vi "UI Main.vi"() -> ()   [LabVIEW 2025]
uses:
  support/User Event - Stop/User Event - Stop.lvlib
  controls/UI Data.ctl
  support/Message Queue/Message Queue.lvlib
  Globals/Global - All UI Loop Stop.vi
  Globals/Global - Configuration Options.vi
  controls/Control State.ctl
  controls/Raw Values.ctl
  controls/Control Configuration.ctl
  controls/All Control Configuration Values.ctl
  Globals/Global - UI Stream and Variable Connections.vi
  Globals/ALL MCS Registers.vi
  5TR Lab/5TR Lab/Global Variables/cRIO channels Input.vi
  <vilib>/numeric/Random Number (Range) U64.vi
  C:/40T/controls/ProfiBusData.ctl
  controls/Profi address.ctl
  controls/Tempratures.ctl
  controls/Power Meters.ctl
  controls/Unit Temp.ctl
  controls/Main UI.ctl
panel:
  in  "Controller Address 2":string
  in  "Hc0 3":i32(listbox)
  in  "Seek Forward Button":bool
  in  "数据列表 2":enum32{"40TR", "Chiller"}(tab)
  in  "Tab Control 2":T1(tab)
  in  "Cluster":T2
  in  "Cluster 2":T3
  in  "ID_HEATER_Stage_3":bool
  in  "ID_HEATER_Stage_2":bool
  in  "OD_HEATER_Stage_1":bool
  in  "ID_HEATER_Stage_3":bool
  in  "ID_HEATER_Stage_2":bool
  in  "Cluster 3":T4
  in  "AUX Chiller Pump_ 2":bool
  in  "AUX Chiller Pump_1":bool
  in  "Hc0 2":i32(listbox)
  in  "Hc1 2":i32(listbox)
  in  "Forget Password":bool
  in  "Add paramter":bool
  in  "数据列表":enum32{"40TR", "Chiller"}(tab)
  in  "Hc0":i32(listbox)
  in  "Hc1":i32(listbox)
  out "WIKA Temprature Transmitters 2":T5
  out "WIKA Temprature Transmitters":T6
  out "Temp":T7
  out "AO1":dbl
  in  "Cluster 4":cluster{"Play Button":bool, "Pause Button":bool}
  in  "Stop Button 2":bool
  in  "Stop Button":bool
  in  "Main System":T8(tab)
  in  "Power":bool
  in  "New User":bool
  in  "Login":bool
  in  "Account":enum16{"AMTECH", "Admin", "Operator"}(ring)=enum."Admin"
  in  "Password":string
  in  "Name":string
  in  "Tab Control":T9(tab)
  in  "Main Configuration":T10={"Unit Model "="", "Reported by"="", "Test Standard"="", "Tested by"="", "Job Number"="NA", "Test Facility"="40TR-Lab", "Power Supply"="", "Other:    PS"="", "Unit Family"="Package", "Requester"="ENG", "Client "="", "Project"="", "Serial Number"="", "Brand"="", "Manufacturer"="", "Test Type"="Package"}
  out "Performed Tests":string[](array[string])
  in  "Load input parameters":bool
  in  "Start Runing":bool
  out "Refrigrant":sgl=98.71708 format="%#.2f"
  out "Ambient_Temp L 2":sgl=98.71708 format="%#.2f"
  out "Ambient_Temp R 2":sgl=98.71708 format="%#.2f"
  out "Coil":sgl=98.71708 format="%#.2f"
  out "Refrigrant Press Tempratures":T11
  out "Ambient R Grid TEMPERATURE  Grid":T12
  out "Ambient L Grid TEMPERATURE Grid":T13
  out "ON-COIL TEMPERATURE  Grid":T12
  out "OFF-COIL TEMPERATURE Grid":T13
  out "Ambient_Temp L":sgl=98.71708 format="%#.2f"
  out "Ambient_Temp R":sgl=98.71708 format="%#.2f"
  out "Ambient":sgl=98.71708 format="%#.2f"
  in  "Save config":bool
  in  "Pressure":T15(array[cluster])
  in  "Power Meters":cluster{"Profi":T14, "Name":T16}[](array[cluster])
  in  "Tempratures":cluster{"Name":T17, "Profi":T14, "Unit":T18}[][](array[cluster])
  out "Main UI":T19
  in  "chiller lab":T20(tab)
  in  "Exit":bool
  out "Control Input Values Crio1":T21(graph)
  out "Control Output Values":T22(graph)
  out "CPU Usage crio2 (%) 2":dbl(graph)
  out "Low Speed Loop Period (ms)":u32
  out "Control Loop Period (ms)":u32
  out "Largest Contiguous Memory (bytes)":dbl(graph)
  out "CPU Usage crio1 (%)":dbl(graph)
  in  "Stop Control":bool
  in  "Run Control":bool
  in  "Control Configurations":T23[](array[typedef])
  in  "Update Control Configuration":bool
  out "Channel 0 Setpoint":dbl
  out "Channel 1 Setpoint":dbl
  out "Channel 2 Setpoint":dbl
  out "Channel 3 Setpoint":dbl
  in  "Temperature Thresholds":dbl[](array[numeric])
  out "Control INputs Crio2":T24(graph)
  in  "Switch to Safe State":bool
  out "System Status":string
  out "Current Control Mode":u16(ring) items=["Safe State", "Control (PID)"]
  out "Connected?":bool
  in  "Connect to Controller":bool
  in  "Controller Address":string
  # "Sensor O/P Values"
  # "Sensor I/P Readings"
  # "LabVIEW Real-Time Control on CompactRIO (RIO Scan Interface)"
  # "Connection Settings"
  # "R"
  # "L"
  # "ON"
  # "OFF"
  # "Element 0 - Chan 0\nElement 1 - Chan 1\nElement 2 - Chan 2\nElement 3 - Chan 3"
  # "Setpoint changes are sent to the target automatically."
  # "Note: In order to set manual outputs in the control loop, you can force IO values through the NI Distributed System Manager, available by right-clicking the CompactRIO target in the project and choosing Utilities > View in System Manager."
  # "Control Configuration changes are sent to the target when you click \"Update Control Configurations\"."
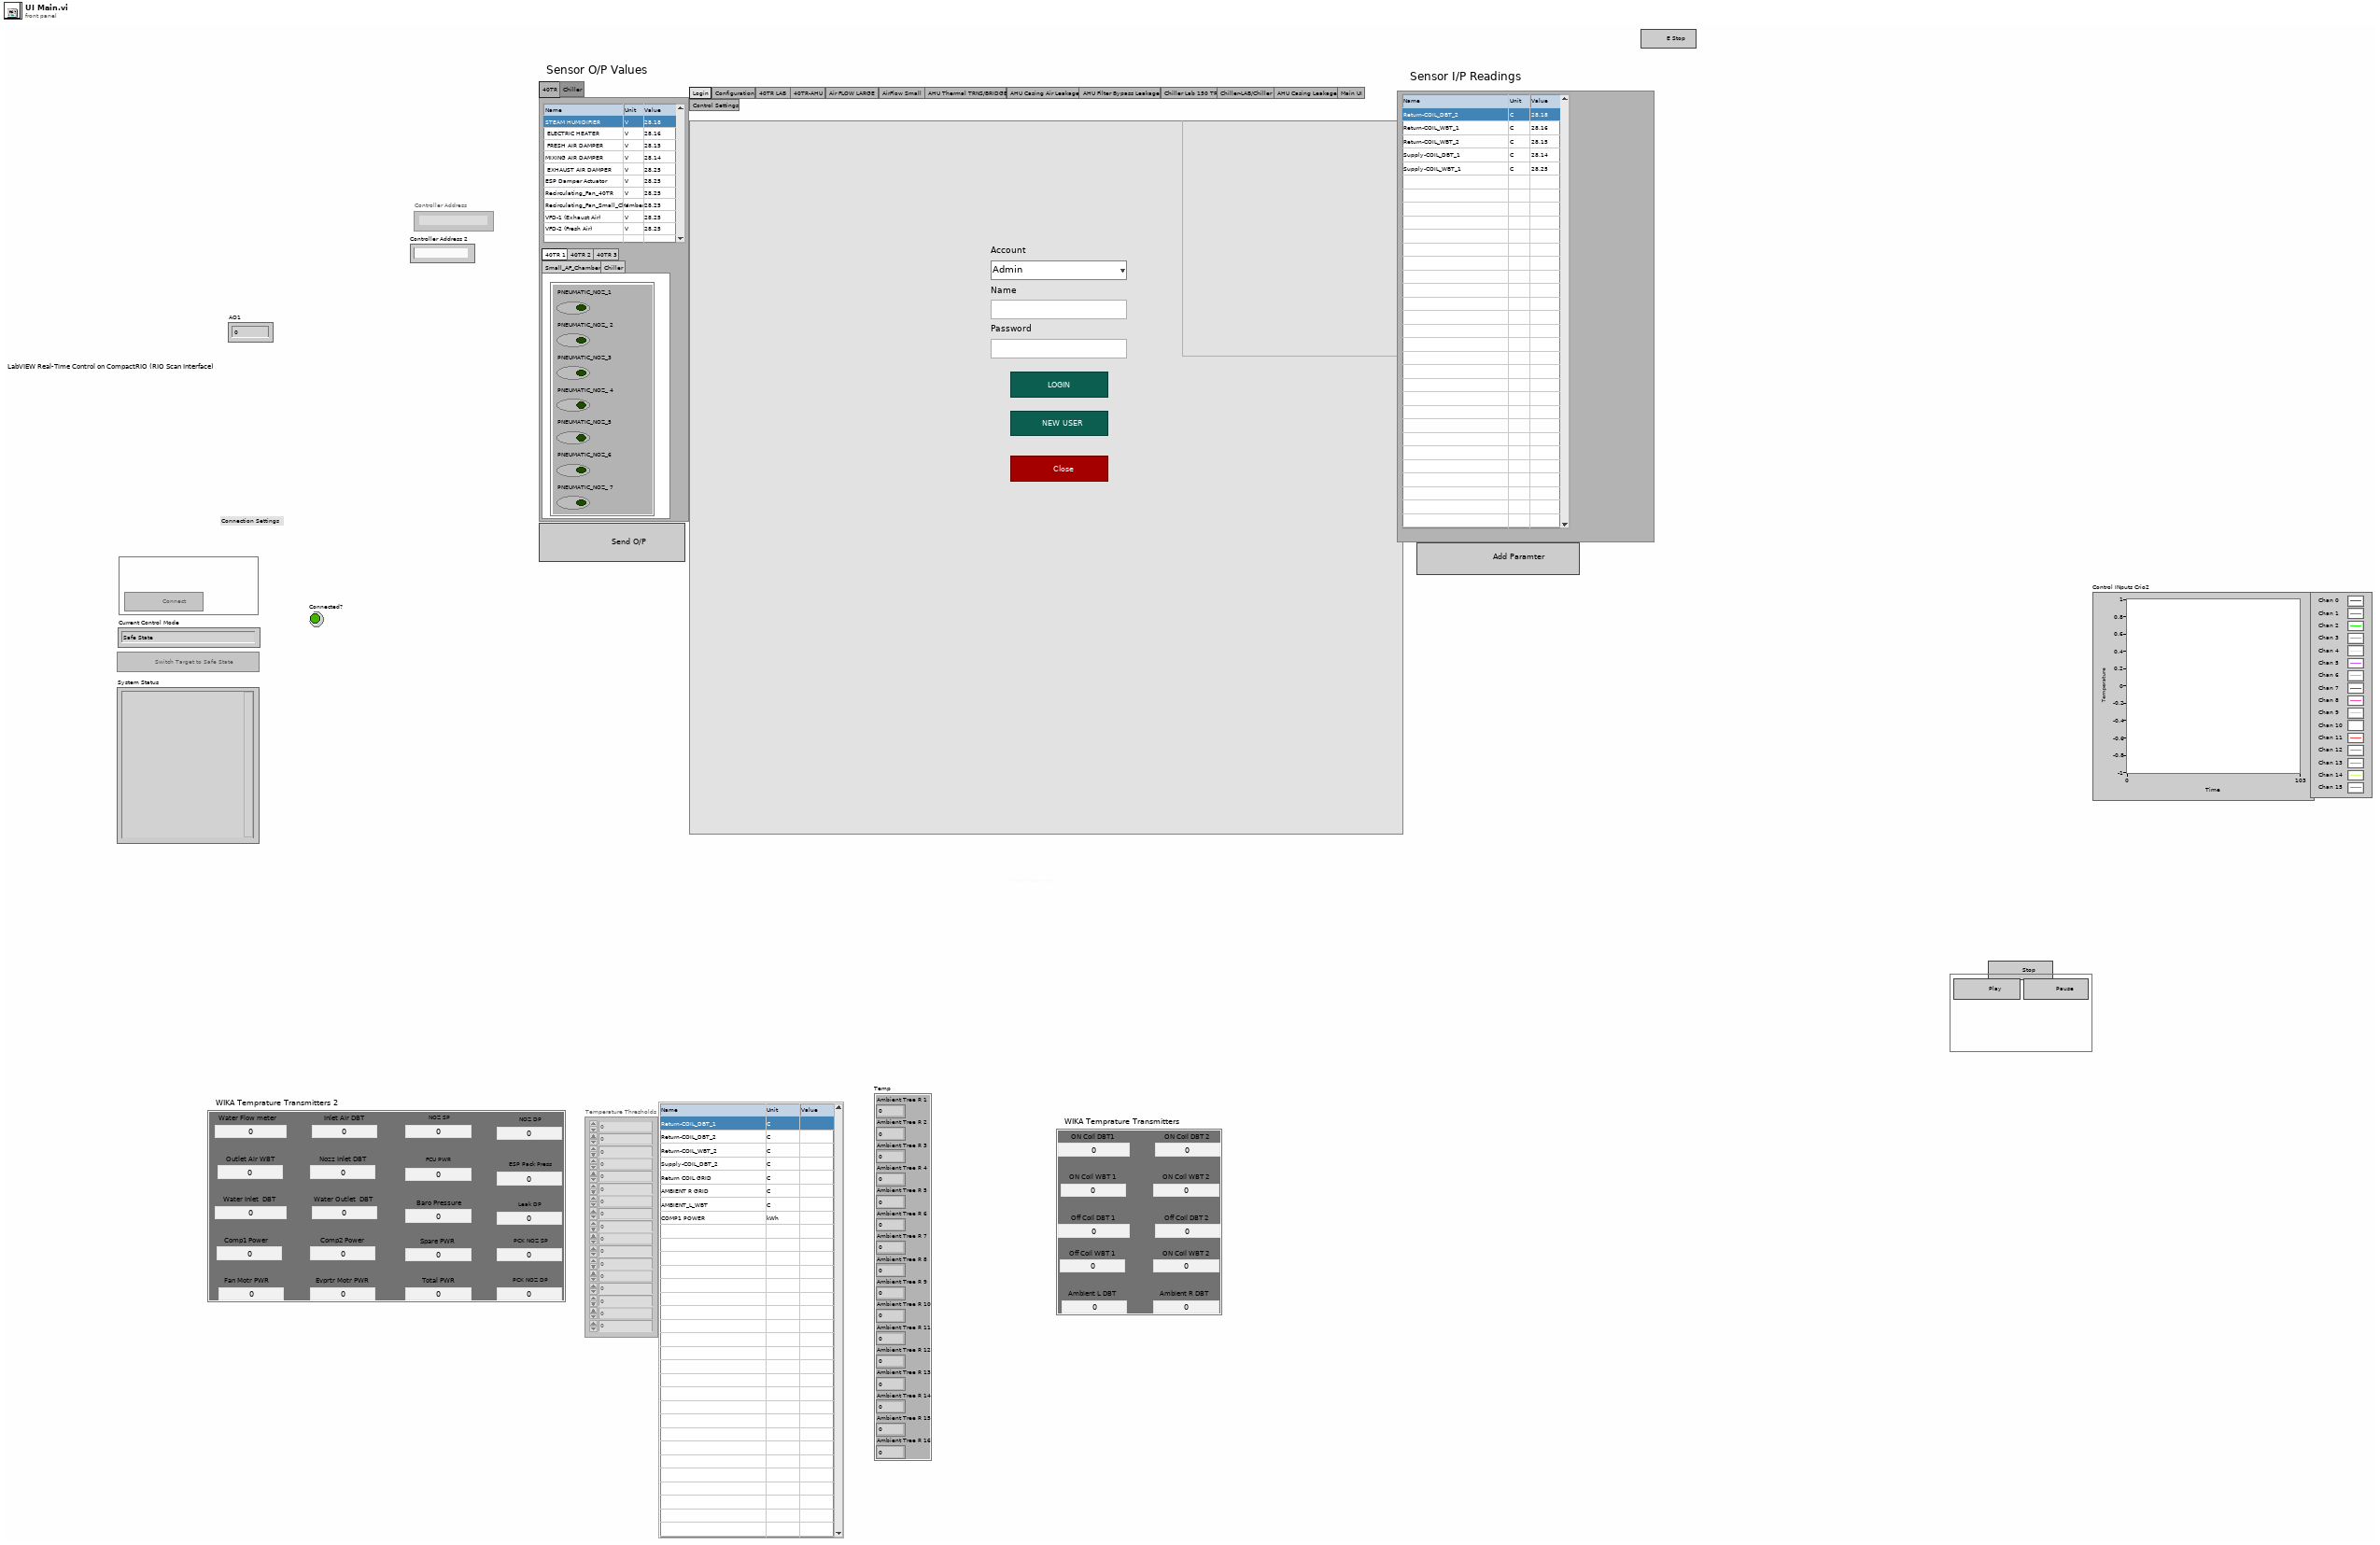
[diagram p1: front panel]
types:
  T1 = enum32{"40TR 1", "40TR 2", "40TR 3", "Small_AF_Chamber", "Chiller"}
  T2 = cluster{"PNEUMATIC_NOZ_1":bool, "PNEUMATIC_NOZ_ 2":bool, "PNEUMATIC_NOZ_3":bool, "PNEUMATIC_NOZ_ 4":bool, "PNEUMATIC_NOZ_5":bool, "PNEUMATIC_NOZ_6":bool, "PNEUMATIC_NOZ_ 7":bool}
  T3 = cluster{"Recirculating_Fan_40TR":bool, "Recirculating_Fan_40TR 2":bool, "STEAM HUMIDIFIER":bool, "VFD-2 (Exahust Air)":bool, "VFD-2 (Fresh Air) ":bool, "VFD_Fan_Leak_setup":bool, "ID_HEATER_Stage_1":bool}
  T4 = cluster{"PNEUMATIC_NOZ_1":bool, "PNEUMATIC_NOZ_ 2":bool, "PNEUMATIC_NOZ_3":bool, "PNEUMATIC_NOZ_ 4":bool, "PNEUMATIC_NOZ_5":bool}
  T5 = cluster{"Water Flow meter":dbl, "Inlet Air DBT ":dbl, "Outlet Air WBT ":dbl, "Nozz Inlet DBT":dbl, "Water Outlet  DBT ":dbl, "Water Inlet  DBT ":dbl, "Comp1 Power":dbl, "Comp2 Power":dbl, "Fan Motr PWR":dbl, "Evprtr Motr PWR":dbl, "Total PWR ":dbl, "Spare PWR":dbl, "Baro Pressure":dbl, "FCU PWR":dbl, "NOZ SP":dbl, "NOZ DP":dbl, "ESP Pack Press":dbl, "Leak DP":dbl, "PCK NOZ SP":dbl, "PCK NOZ DP":dbl}
  T6 = cluster{"ON Coil DBT1  ":dbl, "ON Coil DBT 2":dbl, "ON Coil WBT 1":dbl, "ON Coil WBT 2":dbl, "Off Coil DBT 2":dbl, "Off Coil DBT 1":dbl, "Off Coil WBT 1":dbl, "ON Coil WBT 2":dbl, "Ambient L DBT":dbl, "Ambient R DBT":dbl}
  T7 = cluster{"Ambient Tree R 1":dbl, "Ambient Tree R 2":dbl, "Ambient Tree R 3":dbl, "Ambient Tree R 4":dbl, "Ambient Tree R 5":dbl, "Ambient Tree R 6":dbl, "Ambient Tree R 7":dbl, "Ambient Tree R 8":dbl, "Ambient Tree R 9":dbl, "Ambient Tree R 10":dbl, "Ambient Tree R 11":dbl, "Ambient Tree R 12":dbl, "Ambient Tree R 13":dbl, "Ambient Tree R 14":dbl, "Ambient Tree R 15":dbl, "Ambient Tree R 16":dbl}
  T8 = enum32{"Login", "Configuration", "40TR LAB ", "40TR-AHU", "Air FLOW LARGE", "AirFlow Small ", "AHU Thermal TRNS/BRIDGE", "AHU Casing Air Leakage", "AHU Filter Bypass Leakage ", "Chiller Lab 150 TR", "Chiller-LAB/Chiller", "AHU Casing Leakage", "Main UI", "Control Settings"}
  T9 = enum32{"Input Parameters", "All MCS DATA", "Assigned Sensors Profibus", "Ambient Trees", "Ternds"}
  T10 = cluster{"Unit Model ":string, "Reported by":string, "Test Standard":string, "Tested by":string, "Job Number":string, "Test Facility":string, "Power Supply":string, "Other:    PS":string, "Unit Family":string, "Requester":string, "Client ":string, "Project":string, "Serial Number":string, "Brand":string, "Manufacturer":string, "Test Type":string}
  T11 = cluster{"OFF Coil 1":dbl, "OFF Coil 2":dbl, "OFF Coil 3":dbl, "OFF Coil 4":dbl, "OFF Coil 5":dbl, "OFF Coil 6":dbl, "OFF Coil 7":dbl, "OFF Coil 8":dbl, "OFF Coil 9":dbl, "OFF Coil 10":dbl, "OFF Coil 11":dbl, "OFF Coil 12":dbl, "OFF Coil 13":dbl, "OFF Coil 14":dbl, "OFF Coil 15":dbl, "OFF Coil 16":dbl, "OFF Coil 17":dbl, "OFF Coil 18":dbl, "OFF Coil 19":dbl, "OFF Coil 20":dbl, "OFF Coil 21":dbl, "OFF Coil 22":dbl, "OFF Coil 23":dbl, "OFF Coil 24":dbl, "OFF Coil 25":dbl, "OFF Coil 26":dbl, "OFF Coil 27":dbl, "OFF Coil 28":dbl, "OFF Coil 29":dbl, "OFF Coil 30":dbl, "OFF Coil 31":dbl, "OFF Coil 32":dbl}
  T12 = cluster{"OFF Coil 1":dbl, "OFF Coil 2":dbl, "OFF Coil 3":dbl, "OFF Coil 4":dbl, "OFF Coil 5":dbl, "OFF Coil 6":dbl, "OFF Coil 7":dbl, "OFF Coil 8":dbl, "OFF Coil 9":dbl, "OFF Coil 10":dbl, "OFF Coil 11":dbl, "OFF Coil 12":dbl, "OFF Coil 13":dbl, "OFF Coil 14":dbl, "OFF Coil 15":dbl, "OFF Coil 16":dbl}
  T13 = cluster{"OFF Coil 1":dbl, "OFF Coil 2":dbl, "OFF Coil 3":dbl, "OFF Coil 4":dbl, "OFF Coil 5":dbl, "OFF Coil 6":dbl, "OFF Coil 7":dbl, "OFF Coil 8":dbl, "OFF Coil 9":dbl, "OFF Coil 10":dbl, "OFF Coil 11":dbl, "OFF Coil 12":dbl}
  T14 = typedef "Profi address.ctl" = string
  T15 = cluster{"Profi":T14, "Name":string, "Unit":string}[]
  T16 = typedef "Power Meters.ctl" = string
  T17 = typedef "Tempratures.ctl" = string
  T18 = typedef "Unit Temp.ctl" = string
  T19 = typedef "Main UI.ctl" = cluster{"Baro":dbl, "DBT On Coil":dbl, "WBT On Coil  ":dbl, "DBT Off  Coil ":dbl, "WBT Off Coil    ":dbl, "Noz Tem":dbl, "Noz  SP  49":dbl, "Noz  DP 50":dbl, "Nozzels":cluster{"Noz1":bool, "Noz 2":bool, "Noz 3":bool, "Noz 4":bool, "Noz 5":bool, "Noz 6":bool, "Noz 7":bool}, "ESP":dbl, "ESPDamper":dbl, "Humidifier":dbl, "Ambient Temp":cluster{"L_DBT":dbl, "R_DBT":dbl, "L_WBT":dbl, "R_WBT  ":dbl}, "Nozzels 2":cluster{"Ambient R":bool, "Ambient L":bool}, "Nozzels 3":cluster{"Return":bool}, "Cluster":cluster{"Supply":bool}, "40 TR":dbl, "E Air damper":dbl, "Mixed AD":dbl, "Fresh Air Dammper":dbl, "Nozzels 4":cluster{"VFD 1":dbl, "VFD 2":dbl}, "Nozzels 5":cluster{"OD-Heater1":bool, "OD-Heater 2":bool, "OD-Heater 3":bool}, "Consedate Weight":dbl, "Power Meter":cluster{"Comp1":dbl, "Comp2":dbl, "Cond Fan":dbl, "Ev-Motor":dbl, "Total":dbl, "Spare":dbl}}
  T20 = enum32{"UUT Water LOOP", "Cond -Coils Loop", "AUX Loop ", "Chiller Lab", "Data Monitoring", "System Monitoring"}
  T21 = cluster{"Control Input Values[0]":dbl, "Control Input Values[1]":dbl, "Control Input Values[2]":dbl, "Control Input Values[3]":dbl}
  T22 = cluster{"Control Output Values[0]":dbl, "Control Output Values[1]":dbl, "Control Output Values[2]":dbl, "Control Output Values[3]":dbl}
  T23 = typedef "Control Configuration.ctl" = cluster{"PID Gains":cluster{"proportional gain (Kc)":dbl, "integral gain (Kc*Ts/Ti)":dbl, "derivative gain (Kc*Td/Ts)":dbl}, "Output Range":cluster{"output high":dbl, "output low":dbl}}
  T24 = cluster{"Temperature Values[0]":dbl, "Temperature Values[1]":dbl, "Temperature Values[2]":dbl, "Temperature Values[3]":dbl, "Temperature Values[4]":dbl, "Temperature Values[5]":dbl, "Temperature Values[6]":dbl, "Temperature Values[7]":dbl, "Temperature Values[8]":dbl, "Temperature Values[9]":dbl, "Temperature Values[10]":dbl, "Temperature Values[11]":dbl, "Temperature Values[12]":dbl, "Temperature Values[13]":dbl, "Temperature Values[14]":dbl, "Temperature Values[15]":dbl}
  T25 = enum32{"UUT Water LOOP", "Cond -Coils Loop", "AUX Loop ", "Data Monitoring", "System Monitoring"}
  T26 = enum32{"Control Settings", "Chiller-LAB/Chiller", "40TR LAB ", "Page 2"}
  T27 = typedef "UI Data.ctl" = cluster{"Switch to Safe State Ref":refnum<vi>, "Run Control Ref":refnum<vi>, "Stop Control Ref":refnum<vi>, "Update Control Configurations Ref":refnum<vi>, "Ch 0 Setpoint Ref":refnum<vi>, "Ch 1 Setpoint Ref":refnum<vi>, "Ch 2 Setpoint Ref":refnum<vi>, "Ch 3 Setpoint Ref":refnum<vi>, "Control Configurations Ref":refnum<vi>, "Temperature Thresholds Ref":refnum<vi>}
  T28 = typedef "Message Queue.lvlib/All Message Queues.ctl" = cluster{"UI":refnum<queue>}
  T29 = cluster{"Room DP":dbl, "Barometric Pressure":dbl, "ID Nozzle DP":dbl, "OD Nozzle DP":dbl, "OD UUT Discharge Pressure":dbl, "OD UUT Suction Pressure":dbl, "OD UUT Liquid Pressure":dbl, "ID Humidifier Weight ":dbl, "ID UUT Condensate Weight":dbl, "ID Coil Condensate Weight":dbl, "OD Coil Water flow rate":dbl, "ID Flow Meter Channel":dbl}
  T30 = cluster{"ID UUT inlet DBT":dbl, "ID UUT inlet WBT":dbl, "ID UUT Outlet DBT":dbl, "OD UUT Outlet DBT":dbl, "ID UUT OUTLET WBT":dbl, "OD UUT INLET DBT":dbl, "OD UUT INLET WBT":dbl, "ID_EWT":dbl, "ID_LWT":dbl, "ID_Nozz_Temp":dbl}
  T31 = cluster{"ESP":dbl, "SP":dbl, "DP":dbl, "FCU WFR":dbl, "FCU Water PD":dbl, "RFM (lb/h)":dbl}
  T32 = cluster{"ON Coil 1":dbl, "ON Coil 2":dbl, "ON Coil 3":dbl, "ON Coil 4":dbl, "ON Coil 5":dbl, "ON Coil 6":dbl, "ON Coil 7":dbl, "ON Coil 8":dbl, "ON Coil 9":dbl, "ON Coil 10":dbl, "ON Coil 11":dbl, "ON Coil 12":dbl, "ON Coil 13":dbl, "ON Coil 14":dbl, "ON Coil 15":dbl, "ON Coil 16":dbl}
  T33 = cluster{"Ambient Tree L 1":dbl, "Ambient Tree L 2":dbl, "Ambient Tree L 3":dbl, "Ambient Tree L 4":dbl, "Ambient Tree L 5":dbl, "Ambient Tree L 6":dbl, "Ambient Tree L 7":dbl, "Ambient Tree L 8":dbl, "Ambient Tree L 9":dbl, "Ambient Tree L 10":dbl, "Ambient Tree L 11":dbl, "Ambient Tree L 12":dbl}
  T34 = typedef "Variable References.ctl" = cluster{"CPU Usage":refnum<k21>, "Contiguous Memory":refnum<k21>, "Control Mode":refnum<k21>, "Control Loop Period":refnum<k21>, "Low Speed Loop Period":refnum<k21>, "CPU Usage crio 2":refnum<k21>}
  T35 = typedef "IO References.ctl" = cluster{"Control Input Values":refnum<k21>[], "Control Output Values":refnum<k21>[], "Temperature Values":refnum<k21>[], "Threshold Exceeded":refnum<k21>, "Control Input Values 2":refnum<k21>[], "Control Output Values 2":refnum<k21>[], "Control Digital Values":refnum<k21>[], "Control Digital Values 2":refnum<k21>[]}
  T36 = typedef "Control State.ctl" = enum16{"Safe State", "Control (PID)"}
  T37 = cluster{"Control Input Values crio1 [0]":dbl, "Control Input Values crio1 [1]":dbl, "Control Input Values crio1 [2]":dbl, "Control Input Values crio1 [3]":dbl}
  T38 = cluster{"Input Values Crio2[0]":dbl, "Input Values Crio2[1]":dbl, "Input Values Crio2[2]":dbl, "Input Values Crio2[3]":dbl, "Input Values Crio2[4]":dbl, "Input Values Crio2[5]":dbl, "Input Values Crio2[6]":dbl, "Input Values Crio2[7]":dbl, "Input Values Crio2[8]":dbl, "Input Values Crio2[9]":dbl, "Input Values Crio2[10]":dbl, "Input Values Crio2[11]":dbl, "Input Values Crio2[12]":dbl, "Input Values Crio2[13]":dbl, "Input Values Crio2[14]":dbl, "Input Values Crio2[15]":dbl}
  T39 = typedef "ProfiBusData.ctl" = cluster{"[0]":dbl, "[1]":dbl, "[2]":dbl, "[3]":dbl, "[4]":dbl, "[5]":dbl, "[6]":dbl, "[7]":dbl, "[8]":dbl, "[9]":dbl, "[10]":dbl, "[11]":dbl, "[12]":dbl, "[13]":dbl, "[14]":dbl, "[15]":dbl, "[16]":dbl, "[17]":dbl, "[18]":dbl, "[19]":dbl, "[20]":dbl, "[21]":dbl, "[22]":dbl, "[23]":dbl, "[24]":dbl, "[25]":dbl, "[26]":dbl, "[27]":dbl, "[28]":dbl, "[29]":dbl, "[30]":dbl, "[31]":dbl, "[32]":dbl, "[33]":dbl, "[34]":dbl, "[35]":dbl, "[36]":dbl, "[37]":dbl, "[38]":dbl, "[39]":dbl, "[40]":dbl, "[41]":dbl, "[42]":dbl, "[43]":dbl, "[44]":dbl, "[45]":dbl, "[46]":dbl, "[47]":dbl, "[48]":dbl, "[49]":dbl, "[50]":dbl, "[51]":dbl, "[52]":dbl, "[53]":dbl, "[54]":dbl, "[55]":dbl, "[56]":dbl, "[57]":dbl, "[58]":dbl, "[59]":dbl, "[60]":dbl, "[61]":dbl, "[62]":dbl, "[63]":dbl, "[64]":dbl, "[65]":dbl, "[66]":dbl, "[67]":dbl, "[68]":dbl, "[69]":dbl, "[70]":dbl, "[71]":dbl, "[72]":dbl, "[73]":dbl, "[74]":dbl, "[75]":dbl, "[76]":dbl, "[77]":dbl, "[78]":dbl, "[79]":dbl, "[80]":dbl, "[81]":dbl, "[82]":dbl, "[83]":dbl, "[84]":dbl, "[85]":dbl, "[86]":dbl, "[87]":dbl, "[88]":dbl, "[89]":dbl, "[90]":dbl, "[91]":dbl, "[92]":dbl, "[93]":dbl, "[94]":dbl, "[95]":dbl, "[96]":dbl, "[97]":dbl, "[98]":dbl, "[99]":dbl, "[100]":dbl, "[101]":dbl, "[102]":dbl, "[103]":dbl, "[104]":dbl, "[105]":dbl, "[106]":dbl, "[107]":dbl, "[108]":dbl, "[109]":dbl, "[110]":dbl, "[111]":dbl, "[112]":dbl}
  T40 = cluster{"Message":string, "Message Data":variant}
  T41 = typedef "All Control Configuration Values.ctl" = cluster{"Control State":T36, "Setpoints":T42, "Control Configurations":T23[], "Temperature Thresholds":dbl[]}
  T42 = typedef "Raw Values.ctl" = cluster{"Channel 0":dbl, "Channel 1":dbl, "Channel 2":dbl, "Channel 3":dbl}
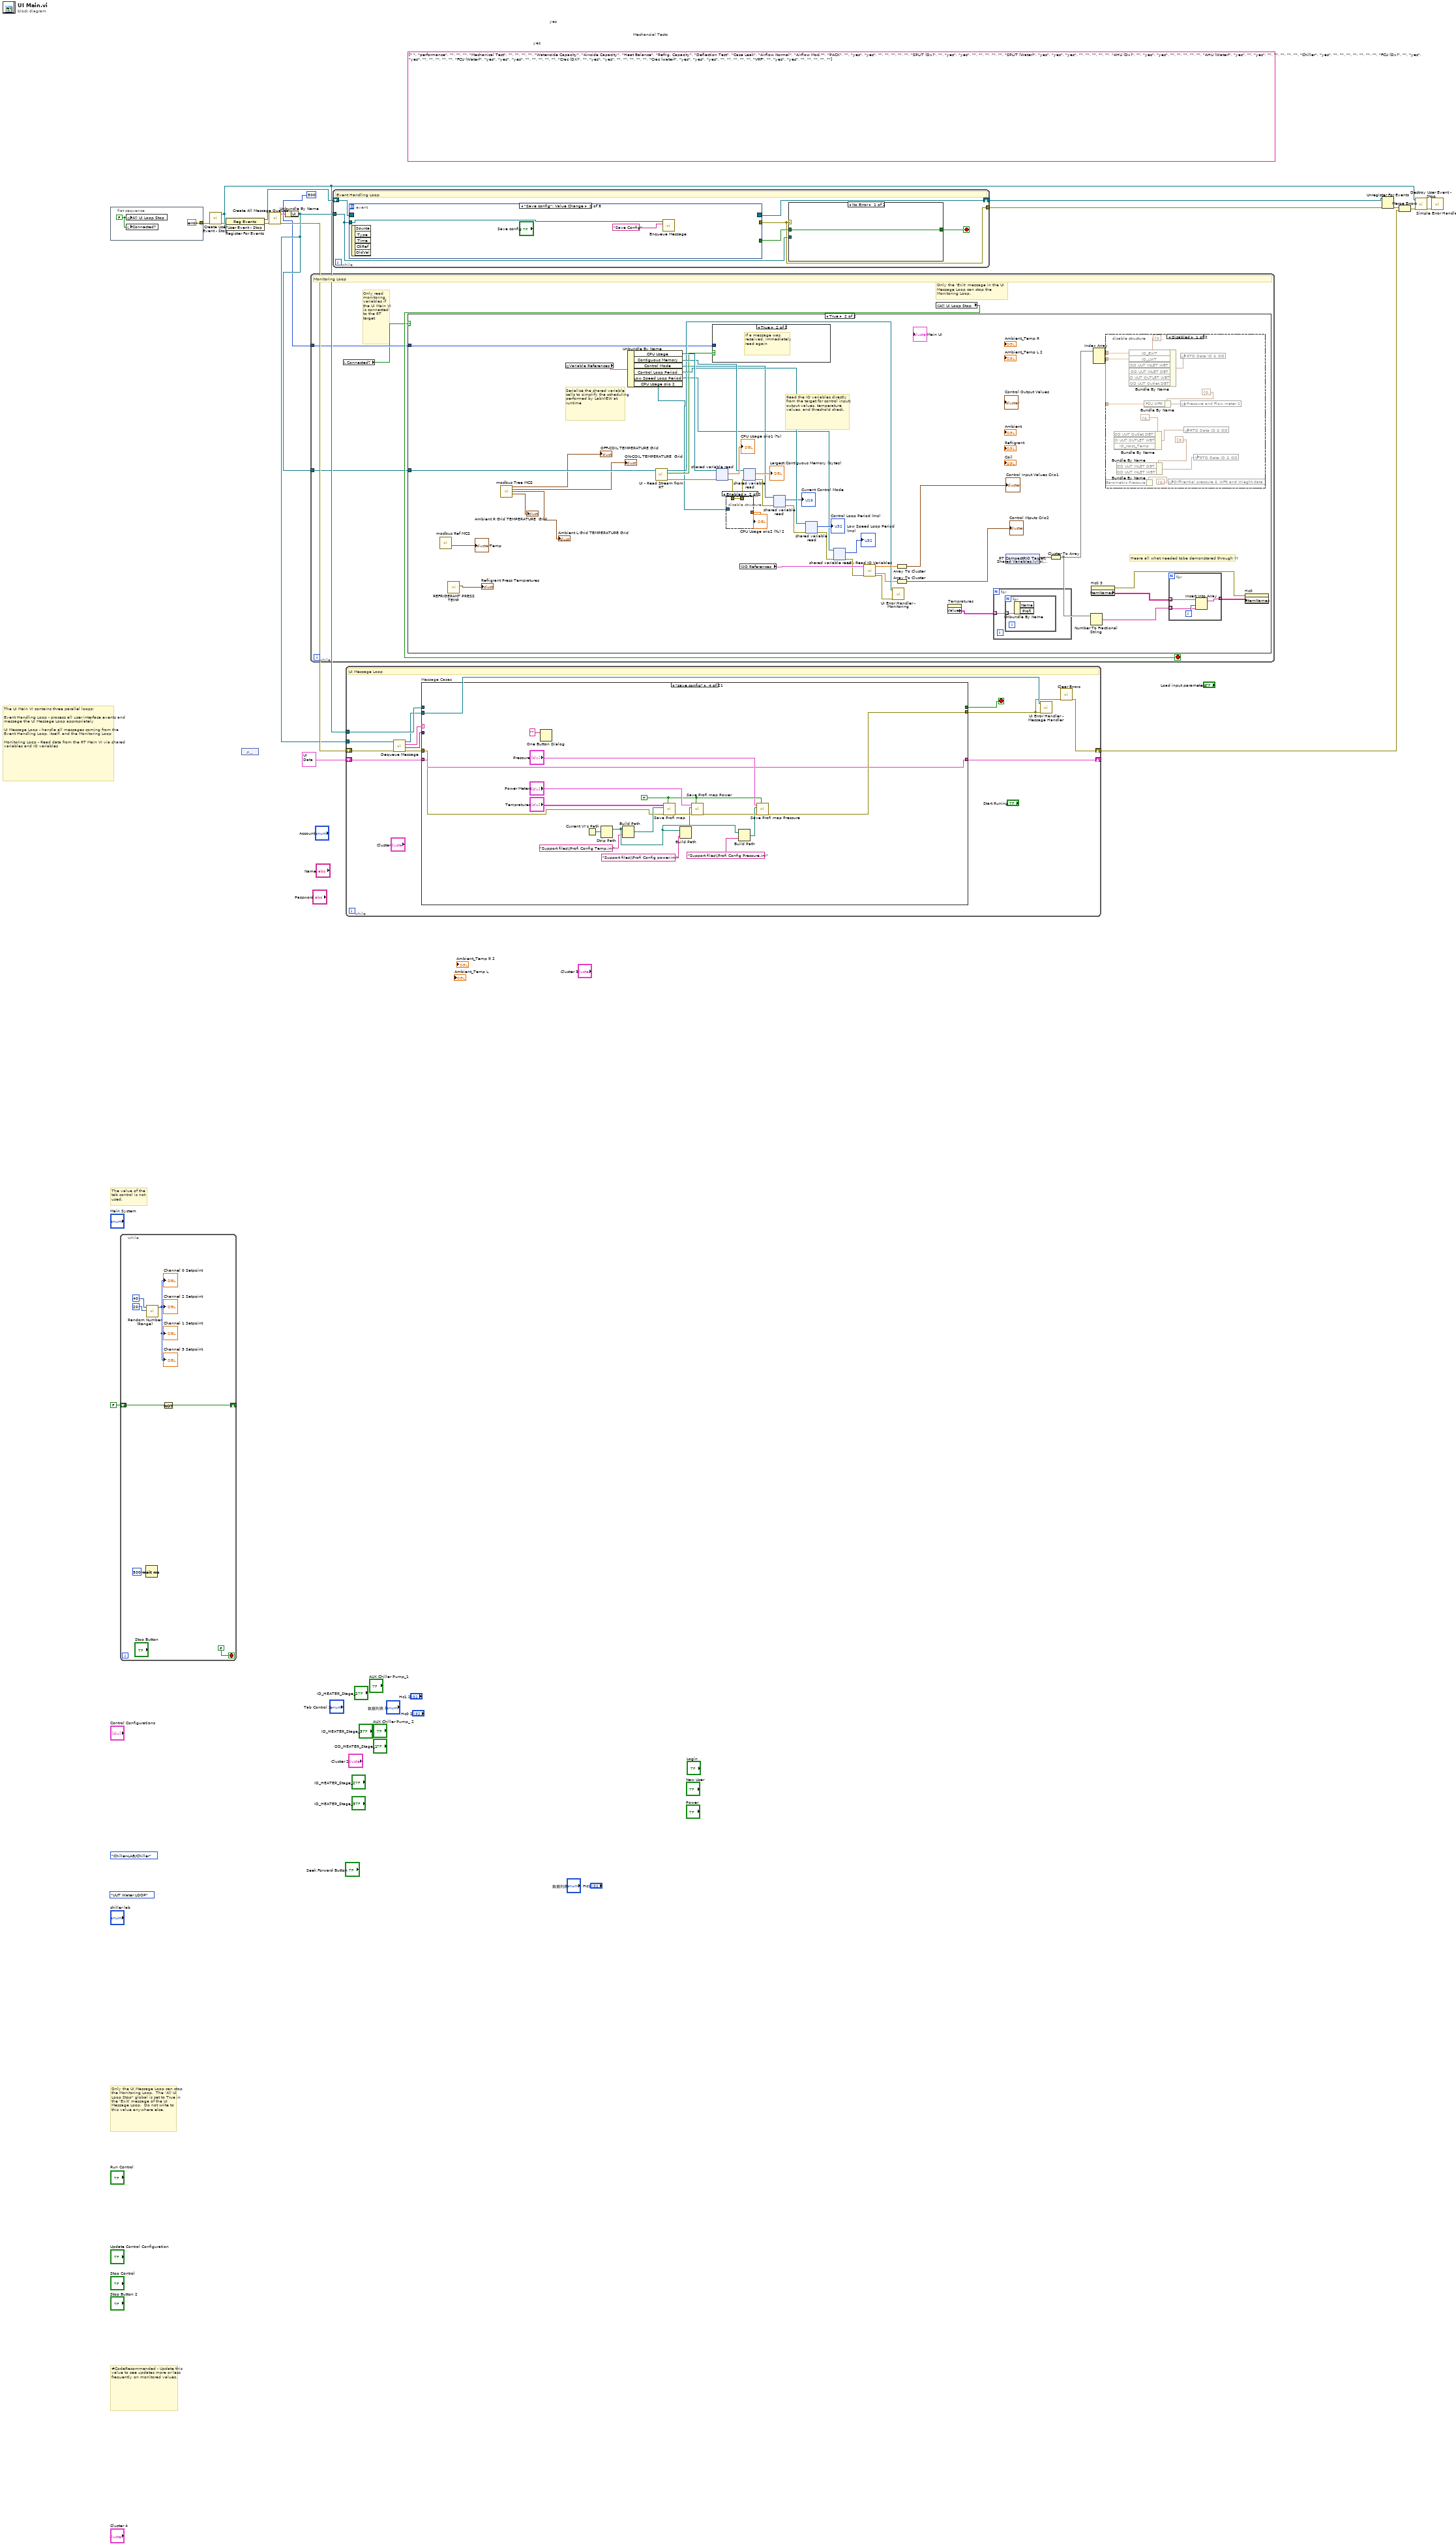
[diagram p0: block diagram]
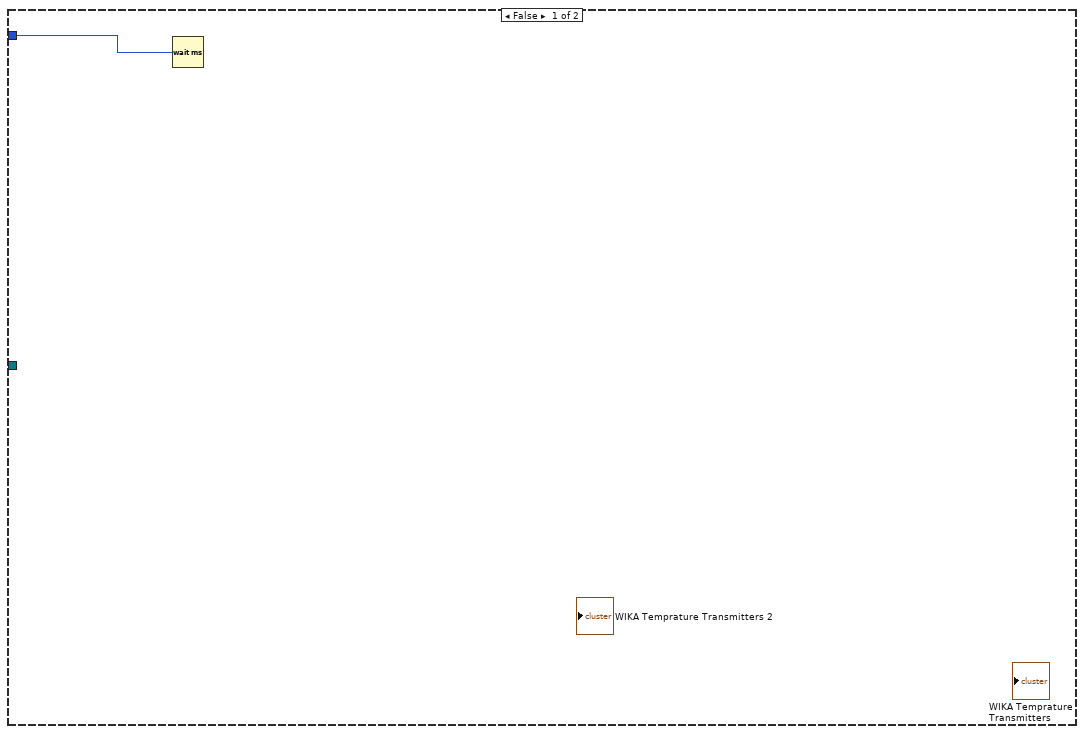
[diagram p2: hidden frame]
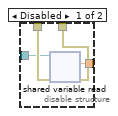
[diagram p4: hidden frame]
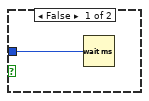
[diagram p5: hidden frame]
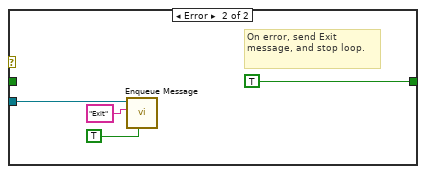
[diagram p6: hidden frame]
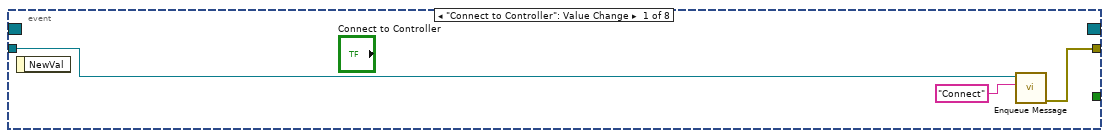
[diagram p7: hidden frame]
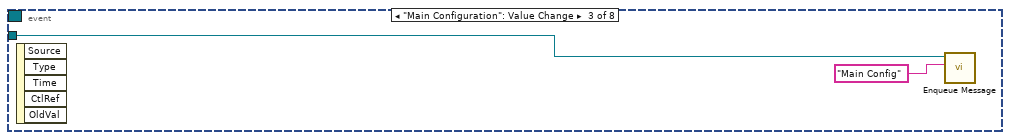
[diagram p8: hidden frame]
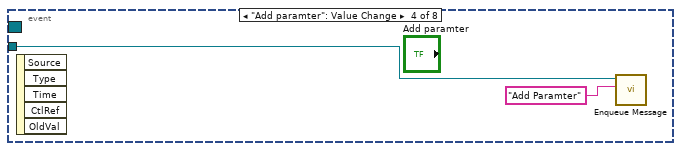
[diagram p9: hidden frame]
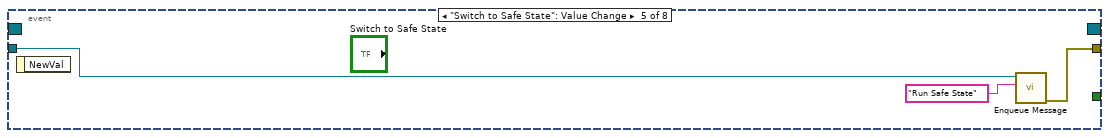
[diagram p10: hidden frame]
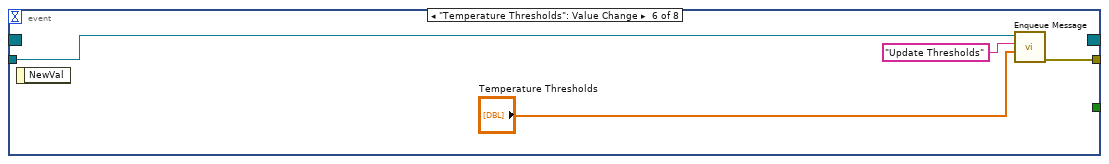
[diagram p11: hidden frame]
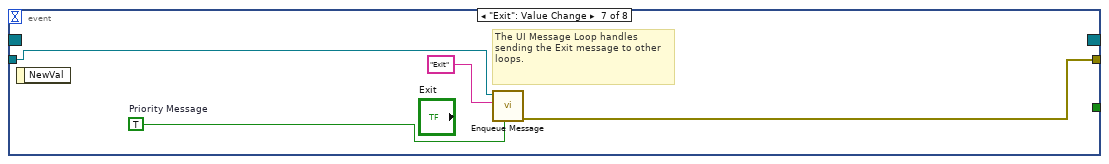
[diagram p12: hidden frame]
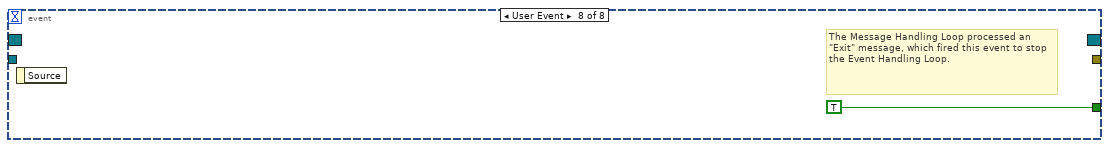
[diagram p13: hidden frame]
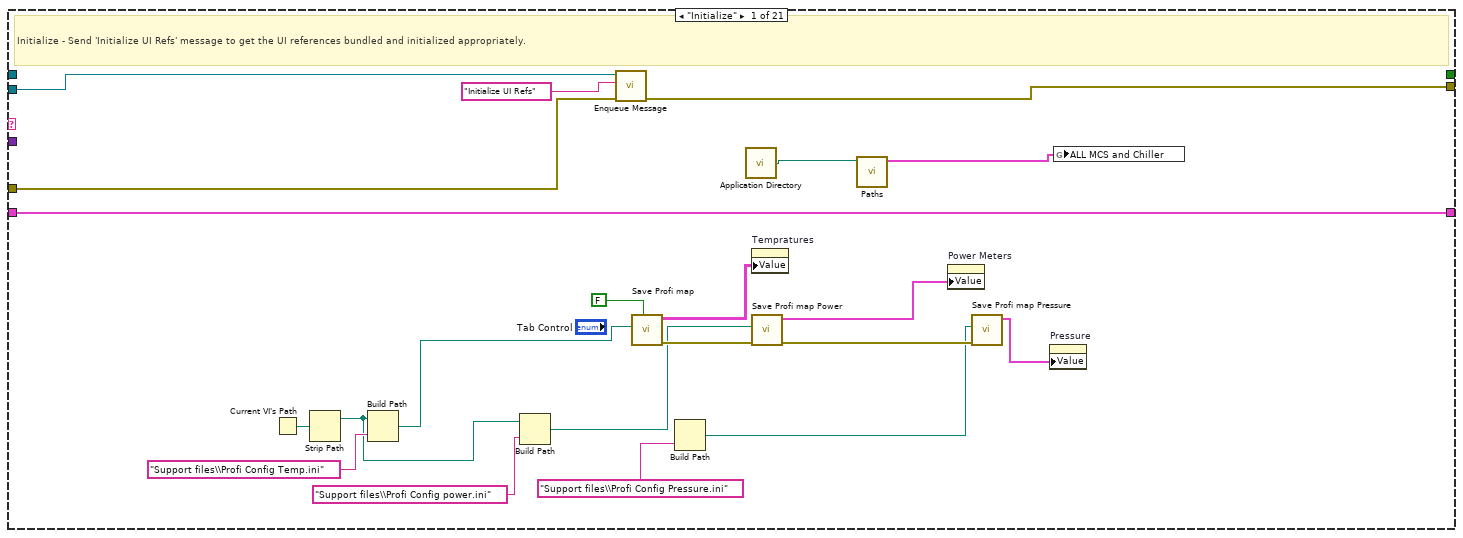
[diagram p14: hidden frame]
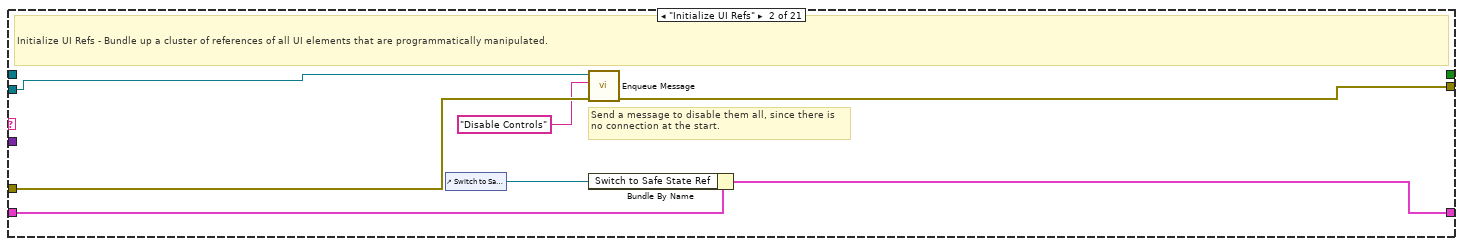
[diagram p15: hidden frame]
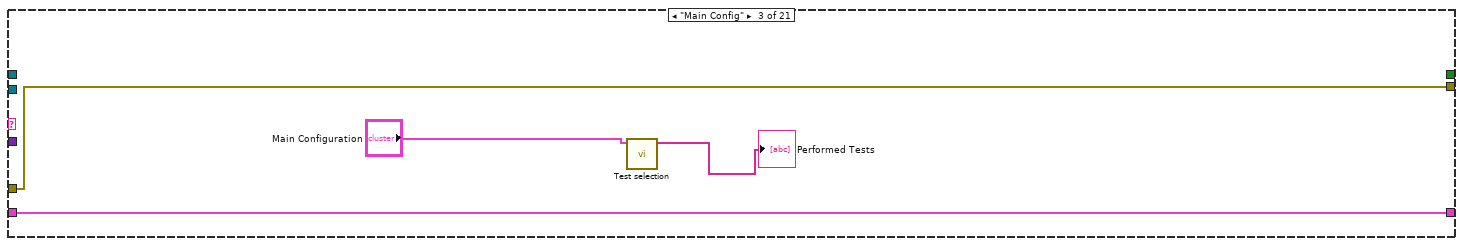
[diagram p16: hidden frame]
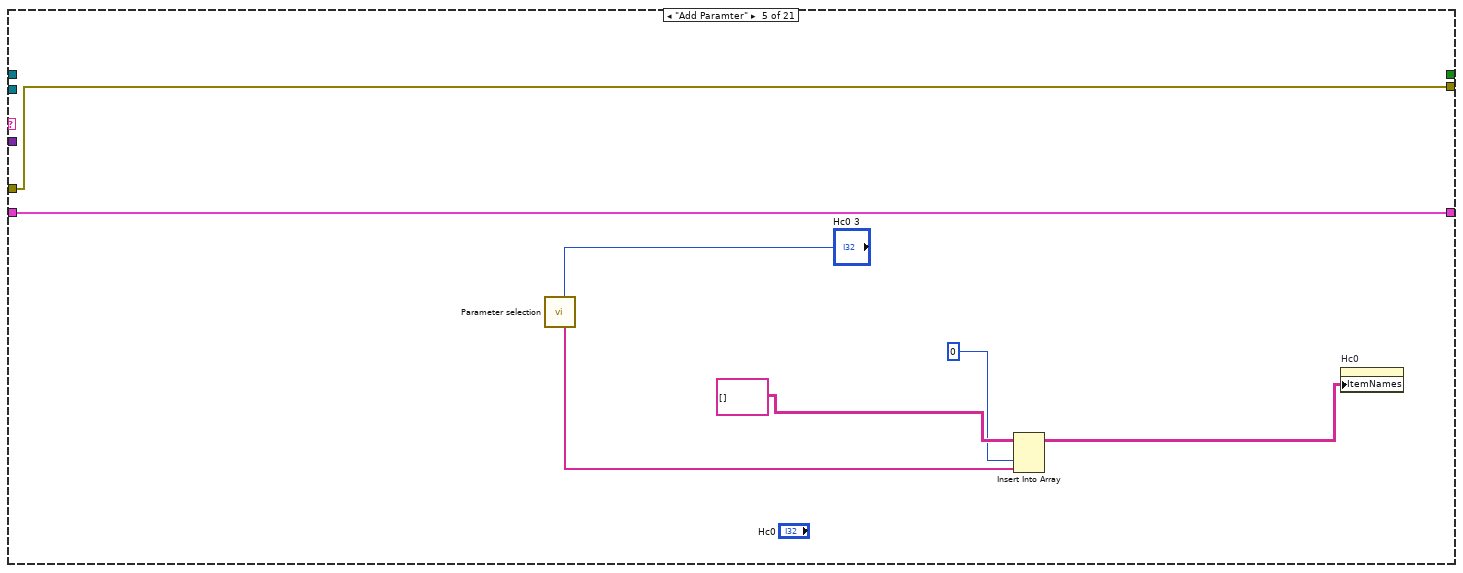
[diagram p17: hidden frame]
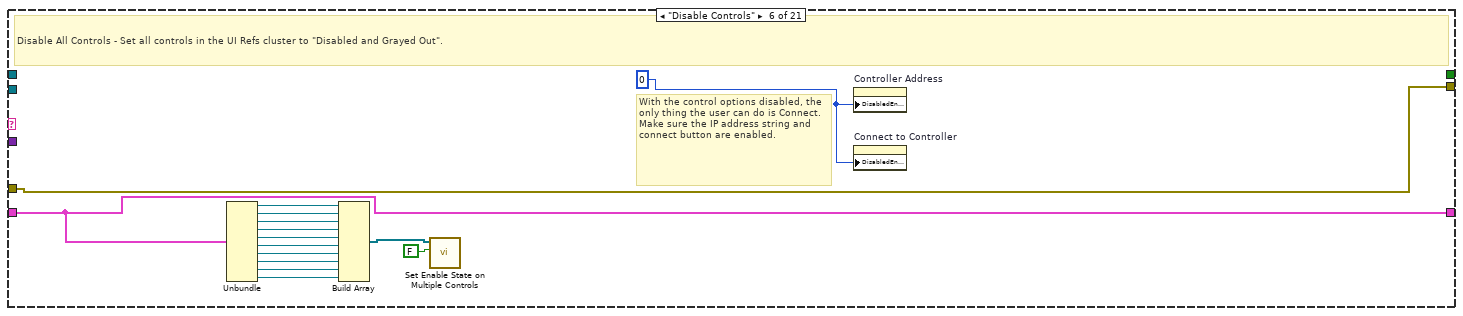
[diagram p18: hidden frame]
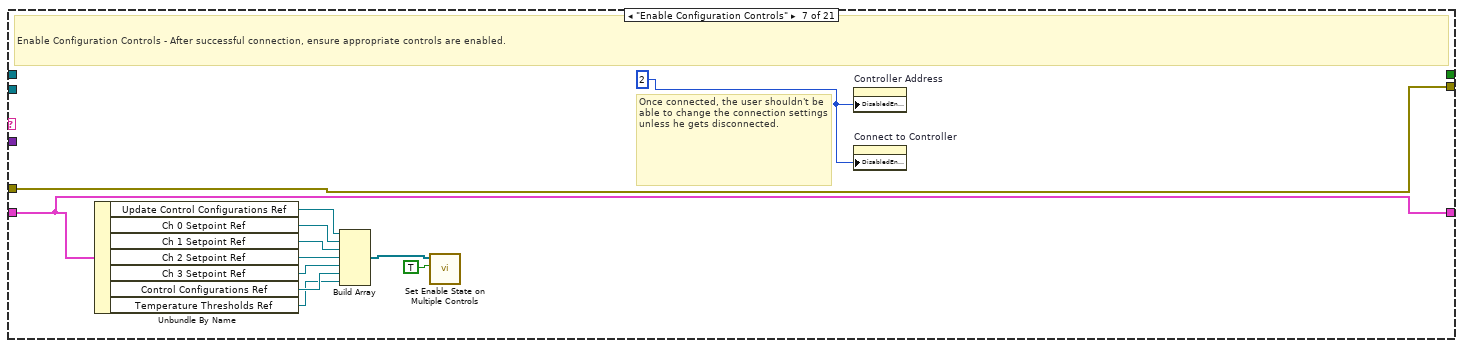
[diagram p19: hidden frame]
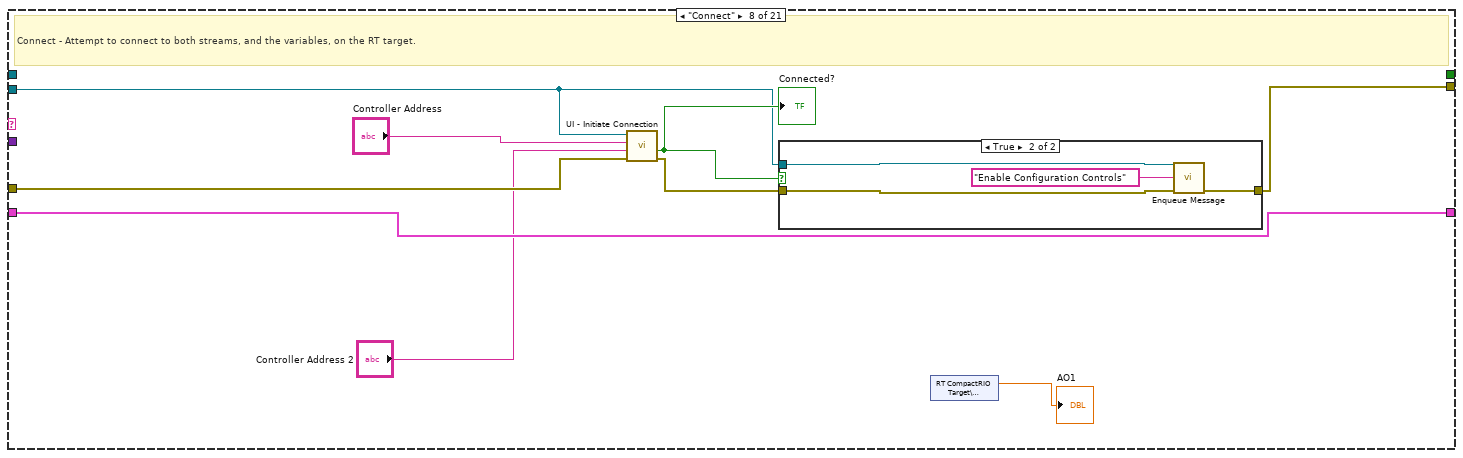
[diagram p20: hidden frame]
diagram:
  (unwired) string[][] [[" ", "performance", "", "", "", "Mechanical Test", "", "", ""], ["", "Water-side Capacity", "Air-side Capacity", "Heat Balance", "Refrig. Capacity", "Deflection Test", "Case Leak", "Airflow Normal", "Airflow Mod.*"], ["PACK", "", "yes", "yes", "", "", "", "", ""], ["SPLIT (Dx)", "", "yes", "yes", "", "", "", "", ""], ["SPLIT (Water)", "yes", "yes", "yes", "", "", "", "", ""], ["AHU (Dx)", "", "yes", "yes", "", "", "", "", ""], ["AHU (Water)", "yes", "", "yes", "", "", "", "", ""], ["Chiller", "yes", "", "", "", "", "", "", ""], ["FCU (Dx)", "", "yes", "yes", "", "", "", "", ""], ["FCU (Water)", "yes", "yes", "yes", "", "", "", "", ""], ["Crac (DX)", "", "yes", "yes", "", "", "", "", ""], ["Crac (water)", "yes", "yes", "yes", "", "", "", "", ""], ["VRF", "", "yes", "yes", "", "", "", "", ""]]
  (unwired) T25."UUT Water LOOP" ("chiller lab")
  (unwired) T26."Chiller-LAB/Chiller" ("Main System")
  # "yes"
  # "yes"
  # "yes"
  # "Mechancial Tests"
  # "#CodeRecommended - Update this value to see updates more or less frequently on monitored values."
  # "The UI Main VI contains three parallel loops:\n\nEvent Handling Loop - process all user interface events and message the UI Message Loop appropriately\n\nUI Message Loop - handle all messages coming from the Event Handling Loop, itself, and the Monitoring Loop\n\nMonitoring Loop - Read data from the RT Main VI via shared variables and IO variables"
  # "The value of the tab control is not used."
  # "Only the UI Message Loop can stop the Monitoring Loop.  The 'All UI Loop Stop\" global is set to True in the 'Exit' message of the UI Message Loop.  Do not write to this value anywhere else."
  n1 = flat-sequence {
    tunnel: [errorcluster {"status"=FALSE, "code"=0, "source"=""} ("error in (no error)")] -> w7
    frame #0 {
      w18 = FALSE
      n2 = global write "Global - All UI Loop Stop.vi" "All UI Loop Stop"(w18) -> ()
      n3 = local write "Connected?"(w18) -> ()
    }
  }
  n4 = while {
    shift-right: [w20] -> _
    shift-left: FALSE ("x") -> [w22]
    stop <- FALSE stop-if-true
    n5 = Wait (ms)(milliseconds to wait=u32 500) -> ()  [unwired: 1 out]
    n6 = call-poly <vilib>:"Random Number (Range).vi"("lower bound (0)"=u64 20, "upper bound (100)"=u64 40) -> ("number"=→"Channel 0 Setpoint" →"Channel 1 Setpoint" →"Channel 2 Setpoint" →"Channel 3 Setpoint":u64)  [unwired: 9 in]
    n7 = Not(x=w22) -> (.not. x?=w20:bool)
  }
  n8 = call "Create User Event - Stop.vi"("error in (no error)"=w7) -> ("error out"=w5:errorcluster, "User Event - Stop"=w2:refnum<user-event>)  [unwired: 9 in]
  n9 = register-events(error in=w5, w2) -> (reference out=w3:refnum<event-registration>, error out=w4:errorcluster)  [unwired: 1 in]
  n10 = control-ref of="Temperature Thresholds"() -> ()  [unwired: 1 out]
  n11 = call "Create All Message Queues.vi"("error in (no error)"=w4) -> ("error out"=w13:errorcluster, "Message Queues out"=w14:T28)  [unwired: 9 in]
  n12 = Unbundle By Name(w14) -> ("UI"=w8:refnum<queue>)
  n13 = while {
    tunnel: w8 -> [w29]
    tunnel: u32 500 ("milliseconds to wait") -> [w28]
    stop <- w30 stop-if-true
    # "Only read monitoring variables if the UI Main VI is connected to the RT target"
    # "Only the 'Exit' message in the UI Message Loop can stop the Monitoring Loop."
    # "Monitoring Loop"
    n14 = local read "Connected?"() -> (w27:bool)
    n15 = case shown="True" w27 {
      tunnel: w29 -> [_ w69]
      tunnel: w28 -> [w31 w64]
      frame False {
        n16 = Wait (ms)(milliseconds to wait=w31) -> ()  [unwired: 1 out]
      }
      frame True {
        # "Heare all what needed tobe demonstared through YI"
        # "Read the IO variables directly from the target for control input/output values, temperature values, and threshold check."
        # "Serialize the shared variable calls to simplify the scheduling performed by LabVIEW at runtime"
        n17 = call "modbus Ref MCS .vi"() -> ("Temp"=→"Temp":T7)  [unwired: 13 in, 2 out]
        n18 = call "REFRIGERANT PRESS TEMP.vi"() -> ("Refrigrant Press Tempratures"=→"Refrigrant Press Tempratures":T11)  [unwired: 10 in, 1 out]
        n19 = call "modbus Tree MCS.vi"() -> ("OFF-COIL"=→"OFF-COIL TEMPERATURE Grid":T13, "ON-COIL"=→"ON-COIL TEMPERATURE  Grid":T32, "Ambietent Left"=→"Ambient L Grid TEMPERATURE Grid":T33, "Ambient Right"=→"Ambient R Grid TEMPERATURE  Grid":T7)  [unwired: 12 in]
        n20 = global read "Global - UI Stream and Variable Connections.vi" "Variable References"() -> (w67:T34)
        n21 = Unbundle By Name(w67) -> ("CPU Usage"=w74:refnum<k21>, "Contiguous Memory"=w73:refnum<k21>, "Control Mode"=w59:refnum<k21>, "Control Loop Period"=w72:refnum<k21>, "Low Speed Loop Period"=w62:refnum<k21>, "CPU Usage crio 2"=w50:refnum<k21>)
        n22 = call "UI - Read Stream from RT.vi"("Message Queue"=w69) -> ("error out"=w71:errorcluster, "Message Received?"=w65:bool, "dup Message Queue"=w68:refnum<queue>)  [unwired: 8 in]
        n23 = case shown="True" w65 {
          tunnel: w64 -> [w101 _]
          frame False {
            n24 = Wait (ms)(milliseconds to wait=w101) -> ()  [unwired: 1 out]
          }
          frame True {
            # "If a message was received, immediately read again"
          }
        }
        n25 = shared-variable-read(w74, w71) -> (w52:errorcluster, →"CPU Usage crio1 (%)":dbl)  [unwired: 2 out]
        n26 = disable-structure shown="Enabled" {
          disable-tunnel: w52 -> [w99 w100]
          disable-tunnel: [w98 w100] -> w51
          disable-tunnel: w50 -> [w97 _]
          disable-tunnel: [w96 _] -> w49
          frame Disabled {
            n27 = shared-variable-read(w97, w99) -> (w98:errorcluster, w96:dbl)  [unwired: 2 out]
          }
          frame Enabled {
          }
        }
        "CPU Usage crio2 (%) 2" <- w49
        n28 = global read "Global - UI Stream and Variable Connections.vi" "IO References"() -> (w58:T35)
        n29 = shared-variable-read(w73, w51) -> (w60:errorcluster, →"Largest Contiguous Memory (bytes)":dbl)  [unwired: 2 out]
        n30 = shared-variable-read(w59, w60) -> (w70:errorcluster, →"Current Control Mode":T36)  [unwired: 2 out]
        n31 = shared-variable-read(w72, w70) -> (w63:errorcluster, →"Control Loop Period (ms)":u32)  [unwired: 2 out]
        n32 = shared-variable-read(w62, w63) -> (w57:errorcluster, →"Low Speed Loop Period (ms)":u32)  [unwired: 2 out]
        n33 = call "UI - Read IO Variables.vi"("IO References"=w58, "error in (no error)"=w57) -> ("Control Input Values crio1"=w55:dbl[], "Input Values Crio2"=w54:dbl[], "error out"=w56:errorcluster)  [unwired: 10 in, 1 out]
        n34 = call "UI Error Handler - Monitoring.vi"("error in (no error)"=w56, "Message Queue"=w68) -> ()  [unwired: 9 in, 1 out]
        n35 = Array To Cluster(array=w55) -> (cluster=→"Control Input Values Crio1":T37)
        n36 = Array To Cluster(array=w54) -> (cluster=→"Control INputs Crio2":T38)
        n37 = property on="Tempratures" class="Arr (strict)"() -> ("Value"=w37:cluster{"Name":T17, "Profi":T14, "Unit":T18}[][])  [unwired: 2 in, 2 out]
        n38 = for {
          tunnel: w37 -> [w90] mode=indexing
          n39 = for {
            tunnel: w90 -> [w91] mode=indexing
            n40 = Unbundle By Name(w91) -> ()  [unwired: 2 out]
          }
        }
        n41 = shared-variable "RT CompactRIO Target\\Shared Variables.lvlib\\Profibus"() -> (w38:T39)  [unwired: 1 in, 1 out]
        n42 = Cluster To Array(cluster=w38) -> (array=w36:dbl[])
        n43 = Number To Fractional String(number=w36) -> (F-format string=w39:string[])  [unwired: 3 in]
        n44 = property on="Hc0 3" class="MCListbox (strict)"() -> (error out=w40:errorcluster, "ItemNames"=w42:string[][])  [unwired: 2 in, 1 out]
        n45 = Index Array(array=w36) -> (element #1=w35:dbl, element #2=w34:dbl, element #3=w33:dbl)  [unwired: 3 in]
        n46 = disable-structure shown="Disabled" {
          disable-tunnel: w35 -> [w85 _]
          disable-tunnel: w34 -> [w84 _]
          disable-tunnel: w33 -> [w83 _]
          frame Disabled {
            n47 = Bundle By Name(cluster=T29 {"Room DP"=0.0, "Barometric Pressure"=0.0, "ID Nozzle DP"=0.0, "OD Nozzle DP"=0.0, "OD UUT Discharge Pressure"=0.0, "OD UUT Suction Pressure"=0.0, "OD UUT Liquid Pressure"=0.0, "ID Humidifier Weight "=0.0, "ID UUT Condensate Weight"=0.0, "ID Coil Condensate Weight"=0.0, "OD Coil Water flow rate"=0.0, "ID Flow Meter Channel"=0.0} ("Diffirential pressure & WFR and Wieght data")) -> ()  [unwired: 1 in, 1 out]
            n48 = Bundle By Name(cluster=T30 {"ID UUT inlet DBT"=0.0, "ID UUT inlet WBT"=0.0, "ID UUT Outlet DBT"=0.0, "OD UUT Outlet DBT"=0.0, "ID UUT OUTLET WBT"=0.0, "OD UUT INLET DBT"=0.0, "OD UUT INLET WBT"=0.0, "ID_EWT"=0.0, "ID_LWT"=0.0, "ID_Nozz_Temp"=0.0} ("RTD Data ID & OD")) -> (w81:T30)  [unwired: 3 in]
            n49 = Bundle By Name(cluster=T30 {"ID UUT inlet DBT"=0.0, "ID UUT inlet WBT"=0.0, "ID UUT Outlet DBT"=0.0, "OD UUT Outlet DBT"=0.0, "ID UUT OUTLET WBT"=0.0, "OD UUT INLET DBT"=0.0, "OD UUT INLET WBT"=0.0, "ID_EWT"=0.0, "ID_LWT"=0.0, "ID_Nozz_Temp"=0.0} ("RTD Data ID & OD")) -> (w80:T30)  [unwired: 2 in]
            n50 = Bundle By Name(cluster=T30 {"ID UUT inlet DBT"=0.0, "ID UUT inlet WBT"=0.0, "ID UUT Outlet DBT"=0.0, "OD UUT Outlet DBT"=0.0, "ID UUT OUTLET WBT"=0.0, "OD UUT INLET DBT"=0.0, "OD UUT INLET WBT"=0.0, "ID_EWT"=0.0, "ID_LWT"=0.0, "ID_Nozz_Temp"=0.0} ("RTD Data ID & OD"), "ID_EWT"=w85, "ID_LWT"=w84) -> (w88:T30)  [unwired: 4 in]
            n51 = Bundle By Name(cluster=T31 {"ESP"=0.0, "SP"=0.0, "DP"=0.0, "FCU WFR"=0.0, "FCU Water PD"=0.0, "RFM (lb/h)"=0.0} ("Pressure and Flow meter 2"), "FCU WFR"=w83) -> (w86:T31)
            n52 = global read "cRIO channels Input.vi" "Diffirential pressure & WFR and Wieght data"() -> ()  [unwired: 1 in]
            n53 = global write "cRIO channels Input.vi" "RTD Data ID & OD"(w88) -> ()
            n54 = global write "cRIO channels Input.vi" "Pressure and Flow meter 2"(w86) -> ()
            n55 = global write "cRIO channels Input.vi" "RTD Data ID & OD"(w81) -> ()
            n56 = global write "cRIO channels Input.vi" "RTD Data ID & OD"(w80) -> ()
          }
          frame Enabled {
          }
        }
        n57 = for {
          tunnel: w42 -> [w95] mode=indexing
          tunnel: [w93] -> w41 mode=indexing
          tunnel: w39 -> [w92] mode=indexing
          i -> [w94]
          n58 = Insert Into Array(array=w95, index=w94, new element=w92) -> (w93:string[])
        }
        n59 = property on="Hc0" class="MCListbox (strict)"(error in=w40, "ItemNames"=w41) -> ()  [unwired: 1 in, 2 out]
      }
    }
    n60 = global read "Global - All UI Loop Stop.vi" "All UI Loop Stop"() -> (w30:bool)
  }
  n61 = while {
    tunnel: w8 -> [w103]
    tunnel: [w105] -> w16
    shift-right: [w102] -> w11
    shift-left: w3 -> [w104]
    stop <- w106 stop-if-true
    # "Event Handling Loop"
    n62 = event shown="[1] \"Save config\": Value Change" {
      selector: w104 -> [_ _ _ _ _ _ _ _]
      dyn-events: [_ _ _ _ _ _ _ _] -> w102
      timeout: _ -> [_ _ _ _ _ _ _ _]
      tunnel: [_ _ _ _ _ _ _ TRUE ("Discard?")] -> w107
      tunnel: w103 -> [w113 w116 w118 w120 w122 w127 w129 _]
      tunnel: [w115 _ _ _ w124 w126 w132 _] -> w105
      event "Connect to Controller": Value Change {
        n63 = event-data() -> ()  [unwired: 1 in, 1 out]
        n64 = call "Enqueue Message.vi"("Message"="Connect", "Message Queue"=w113) -> ("error out"=w115:errorcluster)  [unwired: 8 in, 1 out]
      }
      event "Save config": Value Change {
        n65 = event-data() -> ()  [unwired: 1 in, 5 out]
        n66 = call "Enqueue Message.vi"("Message"="Save Config", "Message Queue"=w116) -> ()  [unwired: 8 in, 2 out]
      }
      event "Main Configuration": Value Change {
        n67 = event-data() -> ()  [unwired: 1 in, 5 out]
        n68 = call "Enqueue Message.vi"("Message"="Main Config", "Message Queue"=w118) -> ()  [unwired: 8 in, 2 out]
      }
      event "Add paramter": Value Change {
        n69 = event-data() -> ()  [unwired: 1 in, 5 out]
        n70 = call "Enqueue Message.vi"("Message"="Add Paramter", "Message Queue"=w120) -> ()  [unwired: 8 in, 2 out]
      }
      event "Switch to Safe State": Value Change {
        n71 = event-data() -> ()  [unwired: 1 in, 1 out]
        n72 = call "Enqueue Message.vi"("Message"="Run Safe State", "Message Queue"=w122) -> ("error out"=w124:errorcluster)  [unwired: 8 in, 1 out]
      }
      event "Temperature Thresholds": Value Change {
        n73 = event-data() -> ()  [unwired: 1 in, 1 out]
        n74 = call "Enqueue Message.vi"("Message Data"="Temperature Thresholds", "Message"="Update Thresholds", "Message Queue"=w127) -> ("error out"=w126:errorcluster)  [unwired: 7 in, 1 out]
      }
      event "Exit": Value Change {
        w130 = TRUE  # Priority Message
        # "The UI Message Loop handles sending the Exit message to other loops."
        n75 = event-data() -> ()  [unwired: 1 in, 1 out]
        n76 = call "Enqueue Message.vi"("Priority Message? (F)"=w130, "Message"="Exit", "Message Queue"=w129) -> ("error out"=w132:errorcluster)  [unwired: 7 in, 1 out]
      }
      event User Event {
        # "The Message Handling Loop processed an \"Exit\" message, which fired this event to stop the Event Handling Loop."
        n77 = event-data() -> ()  [unwired: 1 in, 1 out]
      }
    }
    n78 = case shown="No Error" w105 {
      tunnel: [w108 TRUE ("Discard?")] -> w106
      tunnel: w107 -> [w108 _]
      tunnel: w103 -> [_ w109]
      frame No Error {
      }
      frame Error {
        # "On error, send Exit message, and stop loop."
        n79 = call "Enqueue Message.vi"("Priority Message? (F)"=TRUE ("Discard?"), "Message"="Exit", "Message Queue"=w109) -> ()  [unwired: 7 in, 2 out]
      }
    }
  }
  n80 = while {
    tunnel: w8 -> [w139]
    tunnel: w2 -> [w144]
    shift-right: [w134] -> w17
    shift-left: w13 -> [w143]
    shift-right: [w137] -> _
    shift-left: T27 {"Switch to Safe State Ref"=refnum, "Run Control Ref"=refnum, "Stop Control Ref"=refnum, "Update Control Configurations Ref"=refnum, "Ch 0 Setpoint Ref"=refnum, "Ch 1 Setpoint Ref"=refnum, "Ch 2 Setpoint Ref"=refnum, "Ch 3 Setpoint Ref"=refnum, "Control Configurations Ref"=refnum, "Temperature Thresholds Ref"=refnum} ("Measurement UI Controls") -> [w138]
    stop <- w145 stop-if-true
    # "UI Message Loop"
    n81 = call "Dequeue Message.vi"("error in (no error)"=w143, "Message Queue"=w139) -> ("error out"=w142:errorcluster, "Message Data"=w140:variant, "Message"=w141:string, "dup Message Queue"=w136:refnum<queue>)  [unwired: 6 in]
    n82 = case "Message Cases" shown="\"save config\"" w141 {
      selector: w141 -> [_ _ _ _ _ _ _ _ _ _ _ _ w287 _ w317 _ w352 _ _ _ w414]
      tunnel: w136 -> [w163 w168 _ _ _ _ _ w233 _ w252 _ w269 w288 _ _ _ w356 _ w399 _ _]
      tunnel: w142 -> [w165 w173 w177 w186 w202 w217 w220 w238 w250 w254 w259 w283 w290 w307 w318 w336 w366 w387 w404 w409 _]
      tunnel: [w164 w169 w177 w185 w202 w217 w220 w232 w250 w253 w258 w271 w289 w306 w319 w335 w367 w385 w405 w408 w412] -> w135
      tunnel: [_ _ _ _ _ _ _ _ _ _ _ _ _ _ _ _ _ _ TRUE _ _] -> w145
      tunnel: w140 -> [_ _ _ _ _ _ _ _ _ _ _ w281 _ _ w316 w334 w364 w384 _ _ _]
      tunnel: w144 -> [_ _ _ _ _ _ _ _ _ _ _ _ _ _ _ _ _ _ w403 _ _]
      tunnel: w138 -> [w166 w172 w176 w195 w201 w216 w226 w237 w249 w256 w260 w278 w291 w308 w320 w333 w368 w386 w401 w407 w410]
      tunnel: [w166 w171 w176 w195 w201 w216 w226 w237 w249 w256 w260 w278 w291 w308 w320 w333 w368 w386 w401 w407 w410] -> w137
      frame "Initialize" {
        # "Initialize - Send 'Initialize UI Refs' message to get the UI references bundled and initialized appropriately."
        n83 = Current VI's Path() -> (path=w155:path)
        n84 = Strip Path(path=w155) -> (stripped path=w153:path)  [unwired: 1 out]
        n85 = Build Path(base path=w153, name or relative path="Support files\\Profi Config Temp.ini") -> (appended path=w150:path)
        n86 = Build Path(base path=w153, name or relative path="Support files\\Profi Config power.ini") -> (appended path=w149:path)
        n87 = call "Enqueue Message.vi"("error in (no error)"=w165, "Message"="Initialize UI Refs", "Message Queue"=w163) -> ("error out"=w164:errorcluster)  [unwired: 7 in, 1 out]
        n88 = call "Save Profi map.vi"("Write"=FALSE, "configuration file path"=w150) -> ("error out"=w157:errorcluster, "transposed array"=w147:cluster{"Name":T17, "Profi":T14, "Unit":T18}[][])  [unwired: 8 in]
        n89 = Build Path(name or relative path="Support files\\Profi Config Pressure.ini") -> (appended path=w148:path)  [unwired: 1 in]
        n90 = call <vilib>:"Application Directory.vi"() -> ("Application Directory"=w160:path)
        n91 = property on="Tempratures" class="Arr (strict)"("Value"=w147) -> ()  [unwired: 2 in, 2 out]
        n92 = call "Save Profi map Power.vi"("error in"=w157, "configuration file path"=w149) -> ("error out"=w156:errorcluster, "Array"=w158:cluster{"Sensor":T17, "Profi":T14}[])  [unwired: 8 in]
        n93 = call "Paths.vi"("file path (dialog if empty)"=w160) -> ("All MCS Registers"=w161:cluster{"all rows":string[][]}[])  [unwired: 1 in, 8 out]
        n94 = property on="Power Meters" class="Arr (strict)"("Value"=w158) -> ()  [unwired: 2 in, 2 out]
        n95 = call "Save Profi map Pressure.vi"("configuration file path"=w148, "error in"=w156) -> ("Array"=w146:T15)  [unwired: 7 in, 1 out]
        n96 = property on="Pressure" class="Arr (strict)"("Value"=w146) -> ()  [unwired: 2 in, 2 out]
        n97 = global write "ALL MCS Registers.vi" "ALL MCS and Chiller"(w161) -> ()
      }
      frame "Initialize UI Refs" {
        # "Send a message to disable them all, since there is no connection at the start."
        # "Initialize UI Refs - Bundle up a cluster of references of all UI elements that are programmatically manipulated."
        n98 = control-ref of="Switch to Safe State"() -> (w170:refnum<vi>)
        n99 = call "Enqueue Message.vi"("error in (no error)"=w173, "Message"="Disable Controls", "Message Queue"=w168) -> ("error out"=w169:errorcluster)  [unwired: 7 in, 1 out]
        n100 = Bundle By Name(cluster=w172, "Switch to Safe State Ref"=w170) -> (w171:T27)
      }
      frame "Main Config" {
        n101 = call "Test selection.vi"("Cluster 2"="Main Configuration") -> ("subarray"=→"Performed Tests":string[])  [unwired: 9 in, 1 out]
      }
      frame "save config" {
        w190 = TRUE ("Write")
        n102 = One Button Dialog(message="") -> ()  [unwired: 1 in, 1 out]
        n103 = Current VI's Path() -> (path=w194:path)
        n104 = Strip Path(path=w194) -> (stripped path=w184:path)  [unwired: 1 out]
        n105 = Build Path(base path=w184, name or relative path="Support files\\Profi Config Temp.ini") -> (appended path=w192:path)
        n106 = call "Save Profi map.vi"("Write"=w190, "error in"=w186, "configuration file path"=w192, "Tempratures"="Tempratures") -> ("error out"=w188:errorcluster)  [unwired: 6 in, 1 out]
        n107 = Build Path(base path=w184, name or relative path="Support files\\Profi Config power.ini") -> (appended path=w183:path)
        n108 = call "Save Profi map Power.vi"("Write"=w190, "error in"=w188, "configuration file path"=w183, "Power Meters"="Power Meters") -> ("error out"=w187:errorcluster)  [unwired: 6 in, 1 out]
        n109 = Build Path(base path=w184, name or relative path="Support files\\Profi Config Pressure.ini") -> (appended path=w182:path)
        n110 = call "Save Profi map Pressure.vi"("Pressure"="Pressure", "configuration file path"=w182, "error in"=w187, "Write"=w190) -> ("error out"=w185:errorcluster)  [unwired: 5 in, 1 out]
      }
      frame "Add Paramter" {
        n111 = call "Parameter selection.vi"("Hc0 2"="Hc0 3") -> ("Array 2"=w198:string[])  [unwired: 7 in, 3 out]
        n112 = Insert Into Array(array=string[][] [] ("Item Names"), index (col)=0 ("disabled index (col)"), new element=w198) -> (w199:string[][])  [unwired: 1 in]
        n113 = property on="Hc0" class="MCListbox (strict)"("ItemNames"=w199) -> ()  [unwired: 2 in, 2 out]
      }
      frame "Disable Controls" {
        w204 = 0
        # "With the control options disabled, the only thing the user can do is Connect. Make sure the IP address string and connect button are enabled."
        # "Disable All Controls - Set all controls in the UI Refs cluster to \"Disabled and Grayed Out\"."
        n114 = Unbundle(w216) -> ("Switch to Safe State Ref"=w215:refnum<vi>, "Run Control Ref"=w214:refnum<vi>, "Stop Control Ref"=w213:refnum<vi>, "Update Control Configurations Ref"=w212:refnum<vi>, "Ch 0 Setpoint Ref"=w211:refnum<vi>, "Ch 1 Setpoint Ref"=w210:refnum<vi>, "Ch 2 Setpoint Ref"=w209:refnum<vi>, "Ch 3 Setpoint Ref"=w208:refnum<vi>, "Control Configurations Ref"=w207:refnum<vi>, "Temperature Thresholds Ref"=w203:refnum<vi>)
        n115 = Build Array(w215, w214, w213, w212, w211, w210, w209, w208, w207, w203) -> (w206:refnum<vi>[])
        n116 = call "Set Enable State on Multiple Controls.vi"("Enable?"=FALSE, "Controls"=w206) -> ()  [unwired: 10 in]
        n117 = property on="Controller Address" class="Str"("DisabledEnum"=w204) -> ()  [unwired: 2 in, 2 out]
        n118 = property on="Connect to Controller" class="Bool"("DisabledEnum"=w204) -> ()  [unwired: 2 in, 2 out]
      }
      frame "Enable Configuration Controls" {
        w227 = 2
        # "Once connected, the user shouldn't be able to change the connection settings unless he gets disconnected."
        # "Enable Configuration Controls - After successful connection, ensure appropriate controls are enabled."
        n119 = Unbundle By Name(w226) -> ("Update Control Configurations Ref"=w225:refnum<vi>, "Ch 0 Setpoint Ref"=w224:refnum<vi>, "Ch 1 Setpoint Ref"=w223:refnum<vi>, "Ch 2 Setpoint Ref"=w222:refnum<vi>, "Ch 3 Setpoint Ref"=w221:refnum<vi>, "Control Configurations Ref"=w219:refnum<vi>, "Temperature Thresholds Ref"=w218:refnum<vi>)
        n120 = Build Array(w225, w224, w223, w222, w221, w219, w218) -> (w229:refnum<vi>[])
        n121 = call "Set Enable State on Multiple Controls.vi"("Enable?"=TRUE, "Controls"=w229) -> ()  [unwired: 10 in]
        n122 = property on="Controller Address" class="Str"("DisabledEnum"=w227) -> ()  [unwired: 2 in, 2 out]
        n123 = property on="Connect to Controller" class="Bool"("DisabledEnum"=w227) -> ()  [unwired: 2 in, 2 out]
      }
      frame "Connect" {
        # "Connect - Attempt to connect to both streams, and the variables, on the RT target."
        n124 = call "UI - Initiate Connection.vi"("error in (no error)"=w238, "Controller Address 2"="Controller Address 2", "Controller Address"="Controller Address", "Message Queue"=w233) -> ("error out"=w235:errorcluster, "Connected?"=w234:bool)  [unwired: 6 in]
        "Connected?" <- w234
        n125 = case shown="True" w234 {
          tunnel: w235 -> [w239 w243]
          tunnel: w233 -> [_ w242]
          tunnel: [w239 w241] -> w232
          frame False {
          }
          frame True {
            n126 = call "Enqueue Message.vi"("error in (no error)"=w243, "Message"="Enable Configuration Controls", "Message Queue"=w242) -> ("error out"=w241:errorcluster)  [unwired: 7 in, 1 out]
          }
        }
        n127 = shared-variable "RT CompactRIO Target\\Deterministic Loop Variables.lvlib\\AO1"() -> (→"AO1":dbl)  [unwired: 1 in, 1 out]
      }
      frame "Close Connections" {
        # "Close Connections - Close the connections shared with the Monitoring Loop."
        n128 = local write "Connected?"(FALSE ("Connected?")) -> ()
        n129 = global read "Global - UI Stream and Variable Connections.vi" "Variable References"() -> (w246:T34)
        n130 = global read "Global - UI Stream and Variable Connections.vi" "RT Message Stream"() -> (w247:refnum<k21>)
        n131 = global read "Global - UI Stream and Variable Connections.vi" "IO References"() -> (w244:T35)
        n132 = call "Close Variable Connections.vi"("IO References"=w244, "Variable References"=w246) -> ()  [unwired: 10 in]
        n133 = Destroy Stream Endpoint(11:w247) -> ()  [unwired: 1 in, 1 out]
        n134 = global read "Global - UI Stream and Variable Connections.vi" "UI Command Stream"() -> (w248:refnum<k21>)
        n135 = Destroy Stream Endpoint(11:w248) -> ()  [unwired: 1 in, 1 out]
      }
      frame "Disconnect UI" {
        # "Disconnect UI - Something has gone wrong with the connection. Reinitialize the UI to its disconnected state."
        n136 = local write "Connected?"(FALSE ("Connected?")) -> ()
        n137 = call "Enqueue Message.vi"("error in (no error)"=w254, "Message"="Disable Controls", "Message Queue"=w252) -> ("error out"=w253:errorcluster)  [unwired: 7 in, 1 out]
      }
      frame "Get Control Settings from RT" {
        # "Get Control Settings from RT - Send a command to the RT to retrieve all current control parameter values and send them back to the UI."
        n138 = local read "Connected?"() -> (w257:bool)
        n139 = case shown="True" w257 {
          tunnel: w259 -> [w261 w265]
          tunnel: [w261 w264] -> w258
          frame False {
            # "Don't bother trying to send a message to the RT system if UI Main VI isn't even connected"
          }
          frame True {
            n140 = global read "Global - UI Stream and Variable Connections.vi" "UI Command Stream"() -> (w262:refnum<k21>)
            n141 = shared-variable-write(w262, w265, T40 {"Message"="Send Control Configuration to UI", "Message Data"=variant} ("data in")) -> (w264:errorcluster)  [unwired: 1 in, 2 out]
          }
        }
      }
      frame "Initial UI Values" {
        # "Set values of all setpoint controls via reference."
        # "Initial UI Values - These are the current control values from the RT Control Loop. They are used to initialize the panel of UI Main VI upon successful connection to the RT target."
        n142 = Unbundle By Name(w278) -> ("Ch 0 Setpoint Ref"=w276:refnum<vi>, "Ch 1 Setpoint Ref"=w275:refnum<vi>, "Ch 2 Setpoint Ref"=w274:refnum<vi>, "Ch 3 Setpoint Ref"=w273:refnum<vi>)
        n143 = Build Array(w276, w275, w274, w273) -> (w272:refnum<vi>[])
        n144 = Variant To Data(error in=w283, type=T41 {"Control State"=enum."Safe State", "Setpoints"={"Channel 0"=0.0, "Channel 1"=0.0, "Channel 2"=0.0, "Channel 3"=0.0}, "Control Configurations"=[], "Temperature Thresholds"=[]} ("All FPGA Configuration Values"), Variant=w281) -> (data=w279:T41, error out=w282:errorcluster)
        n145 = Unbundle By Name(w279) -> ("Setpoints"=w277:T42, "Temperature Thresholds"=w266:dbl[], "Control State"=w267:T36)  [unwired: 1 out]
        n146 = local write "Current Control Mode"(w267) -> ()
        n147 = local write "Temperature Thresholds"(w266) -> ()
        n148 = call "Enqueue Message.vi"("error in (no error)"=w282, "Message Data"=w267, "Message"="Update Display Mode", "Message Queue"=w269) -> ("error out"=w271:errorcluster)  [unwired: 6 in, 1 out]
        n149 = Cluster To Array(cluster=w277) -> (array=w268:dbl[])
        n150 = for {
          tunnel: w272 -> [w285] mode=indexing
          tunnel: w268 -> [w284] mode=indexing
          n151 = property class="DigNum"(reference=w285, "Value"=w284) -> ()  [unwired: 1 in, 2 out]
        }
      }
      frame "Run Control", "Run Safe State", "Stop Control" {
        # "Run/Stop buttons - Send a command to switch the RT control loop into the appropriate state. Send a message to update this UI to reflect the new state."
        n152 = local read "Connected?"() -> (w286:bool)
        n153 = case shown="True" w286 {
          tunnel: w290 -> [w292 w302]
          tunnel: [w292 w298] -> w289
          tunnel: w288 -> [_ w297]
          tunnel: w287 -> [_ w296]
          frame False {
            # "Don't bother trying to send a message to the RT system if UI Main VI isn't even connected"
          }
          frame True {
            # "Run Control switches into its respective states. Anything else switches to Safe State."
            n154 = case shown="\"Run Control\"" w296 {
              tunnel: [Control_State."Safe State" ("FPGA State") Control_State."Control (PID)" ("FPGA State")] -> w293
              frame "Run Safe State", "Stop Control", Default {
              }
              frame "Run Control" {
              }
            }
            n155 = global read "Global - UI Stream and Variable Connections.vi" "UI Command Stream"() -> (w294:refnum<k21>)
            n156 = Bundle("Update Control State", "FPGA State"=w293) -> (w299:cluster{string, "FPGA State":T36})  [unwired: 1 in]
            n157 = shared-variable-write(w294, w302, w299) -> (w301:errorcluster)  [unwired: 1 in, 2 out]
            n158 = call "Enqueue Message.vi"("error in (no error)"=w301, "Message Data"=w293, "Message"="Update Display Mode", "Message Queue"=w297) -> ("error out"=w298:errorcluster)  [unwired: 6 in, 1 out]
          }
        }
      }
      frame "Update Control Configuration" {
        # "Update Control Configuration - Send all control configurations to RT."
        n159 = local read "Connected?"() -> (w305:bool)
        n160 = case shown="True" w305 {
          tunnel: w307 -> [w309 w314]
          tunnel: [w309 w313] -> w306
          frame False {
            # "Don't bother trying to send a message to the RT system if UI Main VI isn't even connected"
          }
          frame True {
            w310 = "Update Control Configurations"
            n161 = global read "Global - UI Stream and Variable Connections.vi" "UI Command Stream"() -> (w311:refnum<k21>)
            n162 = Bundle(w310, w310) -> (w312:cluster{string, string})  [unwired: 1 in]
            n163 = shared-variable-write(w311, w314, w312) -> (w313:errorcluster)  [unwired: 1 in, 2 out]
          }
        }
      }
      frame "Update Setpoints", "Update Thresholds" {
        # "Update Setpoints/Thresholds - Send all setpoints/thresholds to RT."
        n164 = local read "Connected?"() -> (w315:bool)
        n165 = case shown="True" w315 {
          tunnel: [w321 w327] -> w319
          tunnel: w318 -> [w321 w325]
          tunnel: w317 -> [_ w324]
          tunnel: w316 -> [_ w323]
          frame False {
            # "Don't bother trying to send a message to the RT system if UI Main VI isn't even connected"
          }
          frame True {
            n166 = global read "Global - UI Stream and Variable Connections.vi" "UI Command Stream"() -> (w322:refnum<k21>)
            n167 = Bundle(w324, "Message Data"=w323) -> (w326:cluster{string, "Message Data":variant})  [unwired: 1 in]
            n168 = shared-variable-write(w322, w325, w326) -> (w327:errorcluster)  [unwired: 1 in, 2 out]
          }
        }
      }
      frame "Update Display Mode" {
        # "Update Display Mode - Enable/Disable Controls appropriately for the new display mode."
        n169 = Unbundle By Name(w333) -> ("Switch to Safe State Ref"=w331:refnum<vi>, "Run Control Ref"=w330:refnum<vi>, "Stop Control Ref"=w329:refnum<vi>)
        n170 = Variant To Data(error in=w336, type=Control_State."Safe State" ("FPGA State"), Variant=w334) -> (data=w332:T36, error out=w335:errorcluster)
        n171 = case shown="\"Control (PID)\"" w332 {
          tunnel: w331 -> [w339 w345]
          tunnel: w330 -> [w337 w346]
          tunnel: w329 -> [w338 w344]
          frame "Control (PID)" {
            n172 = Build Array "Controls to Enable"(w339, w338) -> (w343:refnum<vi>[])
            n173 = Build Array "Controls to Disable"(w337) -> (w341:refnum<vi>[])
            n174 = call "Set Enable State on Multiple Controls.vi"("Enable?"=TRUE, "Controls"=w343) -> ()  [unwired: 10 in]
            n175 = call "Set Enable State on Multiple Controls.vi"("Enable?"=FALSE, "Controls"=w341) -> ()  [unwired: 10 in]
          }
          frame "Safe State", Default {
            # "This frame runs when Control is in Safe State. Only enable the two run buttons."
            n176 = Build Array "Controls to Disable"(w345, w344) -> (w348:refnum<vi>[])
            n177 = Build Array "Controls to Enable"(w346) -> (w350:refnum<vi>[])
            n178 = call "Set Enable State on Multiple Controls.vi"("Enable?"=TRUE, "Controls"=w350) -> ()  [unwired: 10 in]
            n179 = call "Set Enable State on Multiple Controls.vi"("Enable?"=FALSE, "Controls"=w348) -> ()  [unwired: 10 in]
          }
        }
      }
      frame "Critical Error", "Log-Only Error", "Non-Critical Error", "RT Error" {
        # "Error - Display message in status indicator on panel.  If it's a critical error, shut down this VI with an 'Exit' message."
        n180 = case shown="Default" w352 {
          selector: w352 -> [_ w370]
          tunnel: ["UI Error" w370] -> w351
          frame Default {
          }
          frame "RT Error" {
          }
        }
        n181 = Variant To Data(error in=w366, type=errorcluster {"status"=FALSE, "code"=0, "source"=""} ("error constant"), Variant=w364) -> (data=w359:errorcluster, error out=w365:errorcluster)
        n182 = Unbundle By Name(w359) -> ("code"=w358:i32, "source"=w362:string)
        n183 = Format Date/Time String() -> (date/time string=w361:string)  [unwired: 3 in]
        n184 = Format Into String(format string="\n%s: %s %d - %s", w361, w351, w358, w362) -> (resulting string=w353:string)  [unwired: 2 in, 1 out]
        n185 = call "Enqueue Message.vi"("error in (no error)"=w365, "Message Data"=w353, "Message"="Update System Status", "Message Queue"=w356) -> ("error out"=w357:errorcluster, "dup Message Queue"=w355:refnum<queue>)  [unwired: 6 in]
        n186 = case shown="Default" w352 {
          tunnel: w357 -> [w371 w375]
          tunnel: w355 -> [_ w373]
          tunnel: [w371 w374] -> w367
          frame Default {
          }
          frame "Critical Error" {
            n187 = call "Enqueue Message.vi"("error in (no error)"=w375, "Message"="Exit", "Message Queue"=w373) -> ("error out"=w374:errorcluster)  [unwired: 7 in, 1 out]
          }
        }
      }
      frame "Update System Status" {
        # "#CodeRecommended - The code below ensures that the System Status string value does not become too large.  It uses the same maximum size as the RT error log to determine whether or not to remove the last half of the log string. Change this logic if you wish to maintain more/less of the information in the System Status string."
        # "Update System Status - Add a new string to the beginning of the System Status string on the UI."
        n188 = local read "System Status"() -> (w379:string)
        n189 = global read "Global - Configuration Options.vi" "Error Log Max Size (bytes)"() -> (w377:i64)
        n190 = String Length(string=w379) -> (length=w380:i32)
        n191 = Greater?(x=w380, y=w377) -> (0:w378:bool)
        n192 = case shown="True" w378 {
          tunnel: w379 -> [w388 w392]
          tunnel: w377 -> [_ w391]
          tunnel: [w388 w393] -> w376
          frame False {
          }
          frame True {
            n193 = Divide(x=w391, y=i64 2) -> (x/y=w390:dbl)
            n194 = String Subset(string=w392, length (rest)=w390) -> (substring=w393:string)  [unwired: 1 in]
          }
        }
        n195 = Variant To Data(error in=w387, type="", Variant=w384) -> (data=w381:string, error out=w385:errorcluster)
        n196 = Concatenate Strings(w381, w376) -> (→"System Status":string)
      }
      frame "Exit" {
        # "Close all connections"
        # "Stop Monitoring Loop"
        # "Stop Event Handling Loop"
        # "Release the UI Message queue reference"
        # "Stop UI Message Loop"
        # "Exit - Fire the User Event to stop the Event Handling Loop, and toggle the global variable to stop the Monitoring Loop.  This message alone causes all three loops to stop."
        n197 = Release Queue(queue=w399, error in (no error)=w404) -> (error out=w400:errorcluster)  [unwired: 1 in, 2 out]
        n198 = global write "Global - All UI Loop Stop.vi" "All UI Loop Stop"(TRUE ("Stop Monitoring Loop")) -> ()
        n199 = call "Fire User Event - Stop.vi"("User Event - Stop"=w403) -> ("error out"=w402:errorcluster)  [unwired: 10 in]
        n200 = global read "Global - UI Stream and Variable Connections.vi" "Variable References"() -> (w395:T34)
        n201 = global read "Global - UI Stream and Variable Connections.vi" "RT Message Stream"() -> (w396:refnum<k21>)
        n202 = global read "Global - UI Stream and Variable Connections.vi" "IO References"() -> (w394:T35)
        n203 = call "Close Variable Connections.vi"("IO References"=w394, "Variable References"=w395) -> ()  [unwired: 10 in]
        n204 = Destroy Stream Endpoint(11:w396) -> ()  [unwired: 1 in, 1 out]
        n205 = global read "Global - UI Stream and Variable Connections.vi" "UI Command Stream"() -> (w397:refnum<k21>)
        n206 = Destroy Stream Endpoint(11:w397) -> ()  [unwired: 1 in, 1 out]
        n207 = Merge Errors(w402, w400) -> (w405:errorcluster)
      }
      frame "---Copy This Frame---" {
        # "Duplicate this frame when creating new messages.  Change this comment in the duplicated frame to describe this message."
        n208 = Merge Errors(w409) -> (w408:errorcluster)
      }
      frame Default {
        # "'Default' case only runs if there is a message that isn't defined in any of the other cases.  Output a programming error."
        n209 = Format Into String(format string="The invalid message string \"%s\" was received in the Message Handling Loop." ("Invalid Message Loop Message"), w414) -> (resulting string=w411:string)  [unwired: 2 in, 1 out]
        n210 = call <vilib>:"Error Cluster From Error Code.vi"("error message (\"\")"=w411, "error code (0)"=1) -> ("error out"=w412:errorcluster)  [unwired: 7 in]
      }
    }
    n211 = call "UI Error Handler - Message Handler.vi"("error in (no error)"=w135, "Message Queue"=w136) -> ()  [unwired: 9 in, 1 out]
    n212 = call <vilib>:"Clear Errors.vi"("error in (no error)"=w135) -> ("error out"=w134:errorcluster)  [unwired: 5 in, 1 out]
  }
  n213 = Unregister For Events(event registration refnum=w11, error in=w16) -> (error out=w12:errorcluster)
  n214 = Merge Errors(w12, w17) -> (w15:errorcluster)
  n215 = call "Destroy User Event - Stop.vi"("error in (no error)"=w15, "User Event - Stop"=w2) -> ("error out"=w9:errorcluster)  [unwired: 9 in]
  n216 = call <vilib>:"Simple Error Handler.vi"("error in (no error)"=w9) -> ()  [unwired: 4 in, 5 out]
